vi "TS Manager.vi"(11 "notifier":refnum<notifier>) -> ()   [LabVIEW 2025, in "Config Tool.lvlib"]
doc: "This is the main VI for the configuration editor.Copyright 2017 National Instruments Corporation\n\nLicensed under the Apache License, Version 2.0 (the \"License\"); you may not use this file except in compliance with the License. You may obtain a copy of the License at http://www.apache.org/licenses/LICENSE-2.0\nUnless required by applicable law or agreed to in writing, software distributed under the License is distributed on an \"AS IS\" BASIS, WITHOUT WARRANTIES OR CONDITIONS OF ANY KIND, either express or implied. See the License for the specific language governing permissions and limitations under the License."
uses:
  Controls/StateCluster.ctl
  Users/Public/Documents/Sandia National Labs/TSS Plugin/CEF.lvlibp/Repository/CEF_Repository.lvclass
  Users/Public/Documents/Sandia National Labs/TSS Plugin/CEF.lvlibp/Node/NodeRef.ctl
  Users/Public/Documents/Sandia National Labs/TSS Plugin/CEF.lvlibp/Node/CEF_Node.lvclass
  Users/Public/Documents/Sandia National Labs/TSS Plugin/CEF.lvlibp/Node/StandardEvents.ctl
  Controls/FilePaths.ctl
  Users/Public/Documents/Sandia National Labs/TSS Plugin/CEF.lvlibp/glyph manager/glyph manager.ctl
  <vilib>/Utility/config.llb/Config Data RefNum.ctl
  Controls/AddMessage.ctl
  Controls/MoveMessage.ctl
  Users/Public/Documents/Sandia National Labs/TSS Plugin/CEF.lvlibp/hierarchy repo/CEF_HierarchyRepo.lvclass
  Users/Public/Documents/Sandia National Labs/TSS Plugin/System.lvlibp/System/System.lvclass
  Users/Public/Documents/Sandia National Labs/TSS Plugin/CEF.lvlibp/serializable node/CEF_serializable node.lvclass
  ce7dbd15-68e1-444f-b0a0-607e461cde1a.vi
  TestStandUI/Control Globals.vi
  Users/Public/Documents/Sandia National Labs/TSS Plugin/CEF.lvlibp/Node/ReadChildren.vi
  Users/Public/Documents/Sandia National Labs/TSS Plugin/CEF.lvlibp/Node/ReadNodeClass.vi
  Config Tool.lvlib
  Users/Public/Documents/Sandia National Labs/TSS Plugin/CEF.lvlibp
  <vilib>/Utility/config.llb/NI_LVConfig.lvlib
panel:
  in  "Record":bool
  out "Time":dbl format="%<%H:%M:%S>t"
  in  "Initialize Engines":bool
  in  "File Menu":bool
  in  "TreeView":string(tree)="NID741343233"
  in  "ExecutionView Manager":refnum<k7>(container)
  in  "SequenceFileView Manager":refnum<k7>(container)
  in  "Application Manager":refnum<k7>(container)
  in  "Close Executions Btn":refnum<k7>(container)
  in  "Close Sequence File Btn":refnum<k7>(container)
  in  "Open Sequence File Btn":refnum<k7>(container)
  in  "Run Selected Sequence Btn":refnum<k7>(container)
  in  "Entry Point 2 Btn":refnum<k7>(container)
  in  "Entry Point 1 Btn":refnum<k7>(container)
  in  "Executions ComboBox":refnum<k7>(container) caption="Executions"
  in  "Sequences ComboBox":refnum<k7>(container) caption="Sequences"
  in  "Sequence Files ComboBox":refnum<k7>(container) caption="Sequence Files"
  in  "Execution View":refnum<k7>(container)
  in  "Terminate All Btn":refnum<k7>(container)
  in  "Break/Resume Btn":refnum<k7>(container)
  in  "Terminate/Restart Btn":refnum<k7>(container)
  in  "Report Viewer":refnum<k7>(container)
  in  "TS Pane":bool
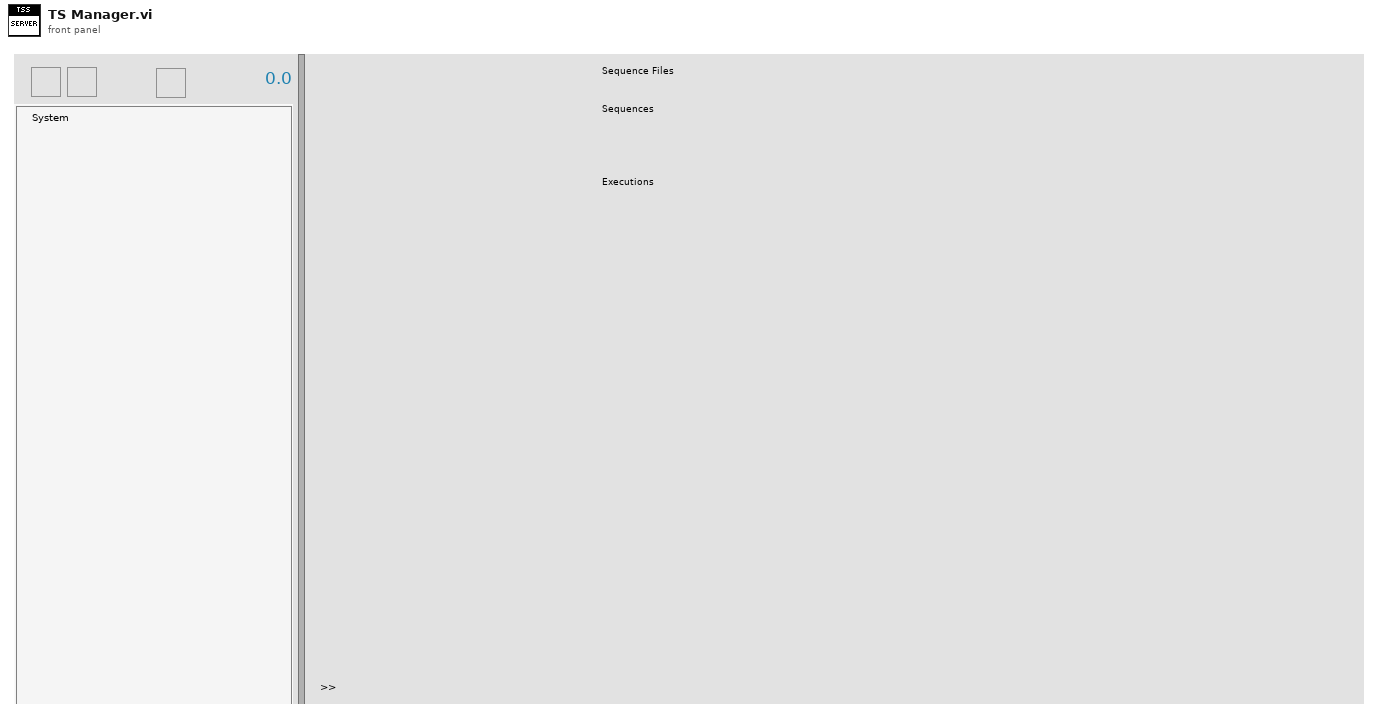
[diagram p1: front panel]
types:
  T1 = typedef "Config Tool.lvlib/StateCluster.ctl" = cluster{"repository":refnum<class "CEF_Repository.lvclass">, "root":T2, "standard events":T3, "paths":T4, "glyph manager":T5, "current path":path, "unsaved changes":bool, "menu":refnum<k9>, "Error Log":refnum<file>, "INI file ref":T6, "Record":bool, "tdms file":refnum<k34>}
  T2 = typedef "CEF.lvlibp/CEF_Node.lvclass/NodeRef.ctl" = refnum<data-value>
  T3 = typedef "CEF.lvlibp/CEF_Node.lvclass/StandardEvents.ctl" = cluster{"user event":refnum<user-event>, "node change":refnum<user-event>, "cache state":refnum<user-event>, "refresh UI":refnum<user-event>, "stop event":refnum<user-event>, "Quit App":refnum<user-event>}
  T4 = typedef "Config Tool.lvlib/FilePaths.ctl" = cluster{"Configuration":path, "Plugin":path, "Glyphs":path, "Data":path, "Error Log":path}
  T5 = typedef "CEF.lvlibp/glyph manager.ctl" = cluster{"search paths":path[], "glyph map":variant, "base glyphs":cluster{"image type":i32, "image depth":i32, "image":u8[], "mask":u8[], "colors":u32[], "Rectangle":cluster{"left":i16, "top":i16, "right":i16, "bottom":i16}}[], "desired overlays":string[]}
  T6 = typedef "NI_LVConfig.lvlib/Config Data RefNum.ctl" = refnum<k1>
  T7 = cluster{"user event":refnum<user-event>, "node change":refnum<user-event>, "cache state":refnum<user-event>, "refresh UI":refnum<user-event>, "stop event":refnum<user-event>, "Quit App":refnum<user-event>}
  T8 = typedef "Config Tool.lvlib/AddMessage.ctl" = cluster{"subNode":string, "Node ID":string}
  T9 = typedef "Config Tool.lvlib/MoveMessage.ctl" = cluster{"node ref":T2, "new parent":T2, "Index":i32}
  T10 = cluster{"Message Name":string, "data string":string}
  T11 = typedef "LVPoint32TypeDef.ctl" = cluster{"Horizontal":i32, "Vertical":i32}
  T12 = cluster{"data name":string, "drag data":variant}[]
  T13 = cluster{"removable":bool, "movable":bool, "duplicate":bool}
  T14 = cluster{"message name":string, "data string":string}
  T15 = enum16{"Start Timer", "Read Time", "Pause", "Resume"}
  T16 = enum16{"open", "open or create", "create or replace", "create", "open (read-only)"}
  T17 = cluster{"search paths":path[], "glyph map":variant, "base glyphs":cluster{"image type":i32, "image depth":i32, "image":u8[], "mask":u8[], "colors":u32[], "Rectangle":cluster{"left":i16, "top":i16, "right":i16, "bottom":i16}}[], "desired overlays":string[]}
  T18 = cluster{"ID":string, "parent ID":string, "node type":string, "text":string, "additional text":string, "glyph":string, "depth":i32, "glyph overlay":string}[]
  T19 = cluster{"ID":string, "parent ID":string, "node type":string, "text":string, "additional text":string, "glyph":string, "depth":i32, "glyph overlay":string}
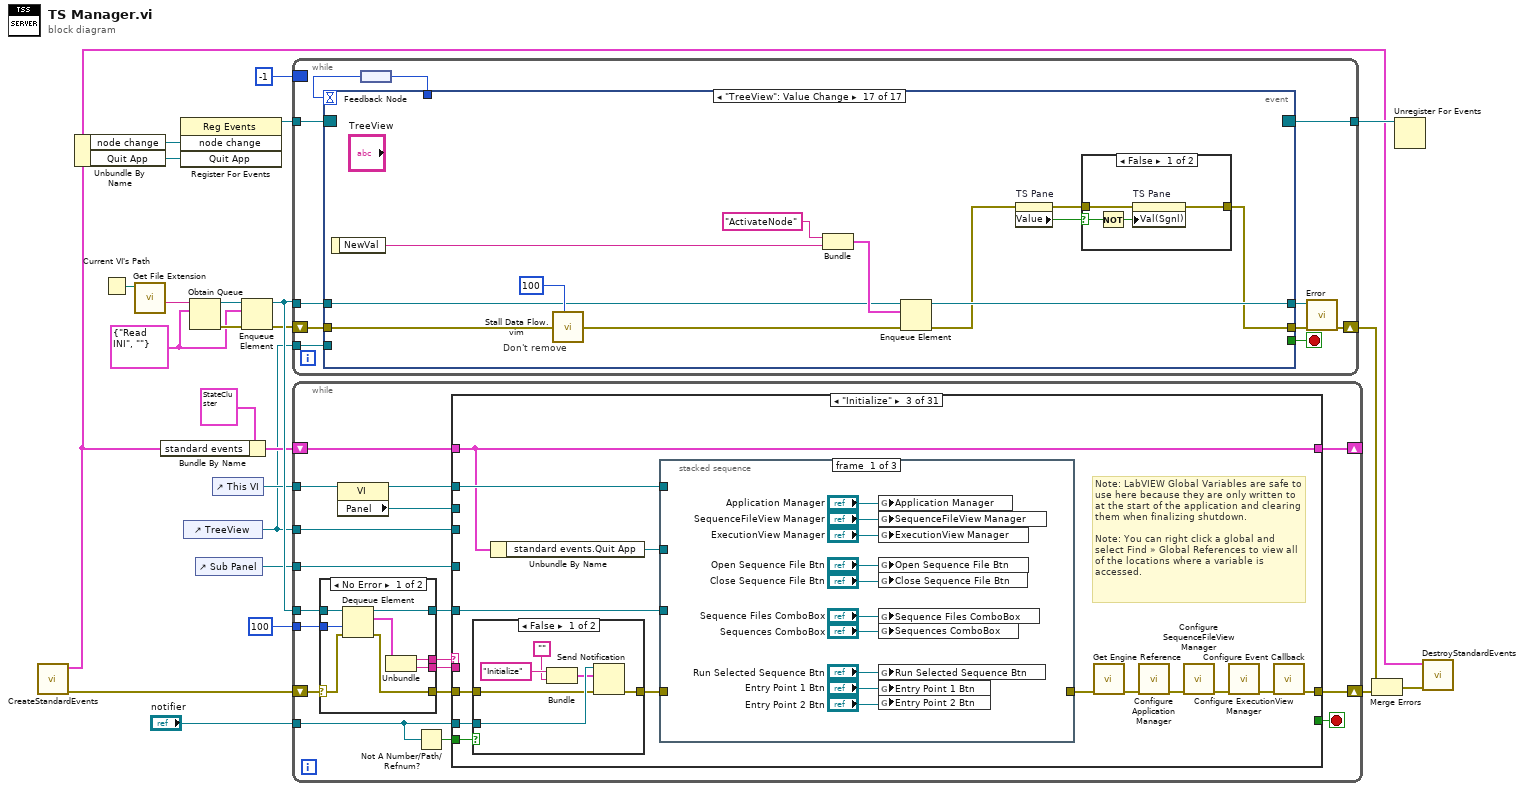
[diagram p0: block diagram]
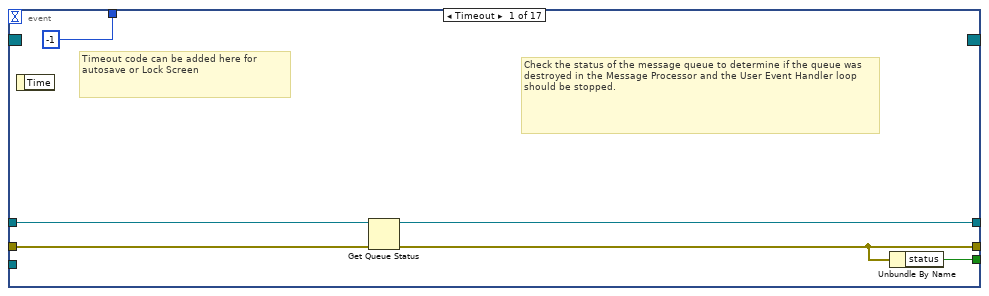
[diagram p2: hidden frame]
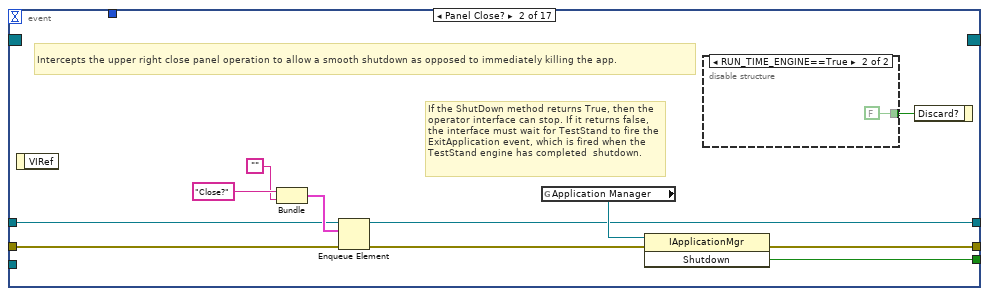
[diagram p3: hidden frame]
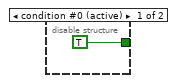
[diagram p4: hidden frame]
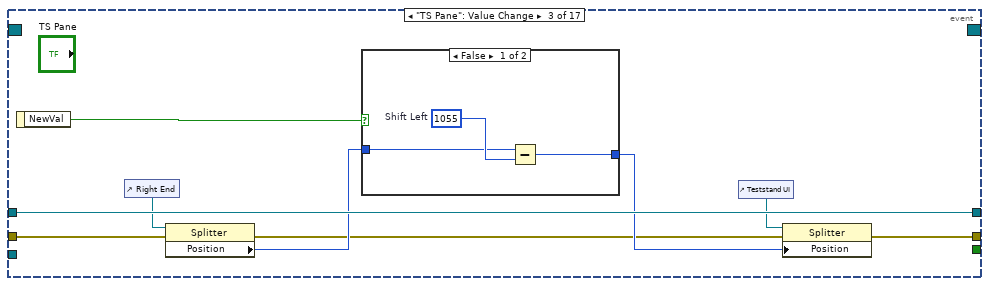
[diagram p5: hidden frame]
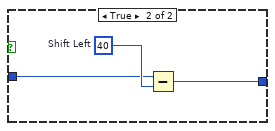
[diagram p6: hidden frame]
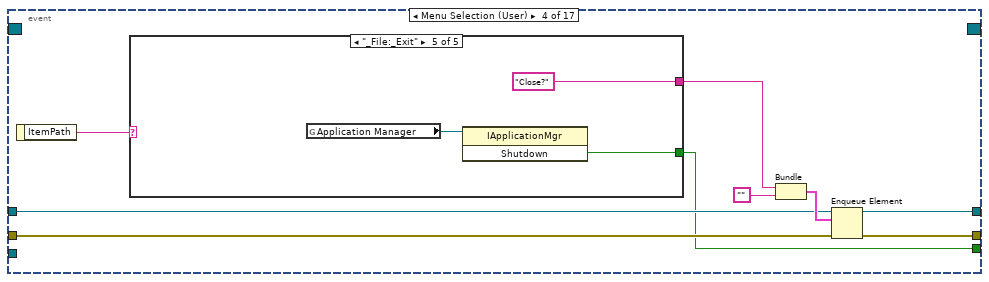
[diagram p7: hidden frame]
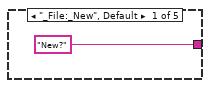
[diagram p8: hidden frame]
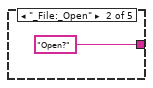
[diagram p9: hidden frame]
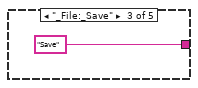
[diagram p10: hidden frame]
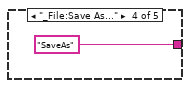
[diagram p11: hidden frame]
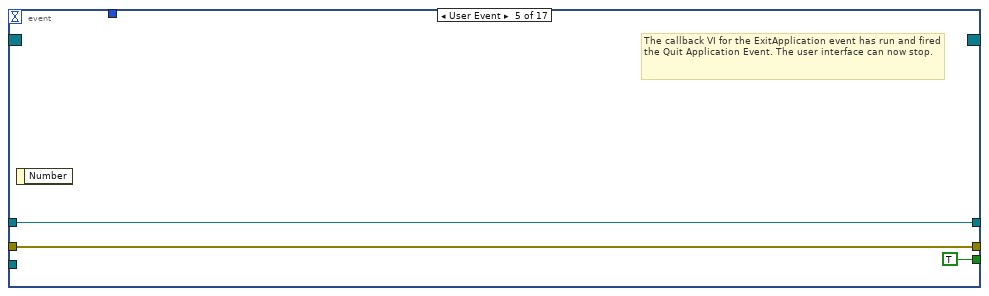
[diagram p12: hidden frame]
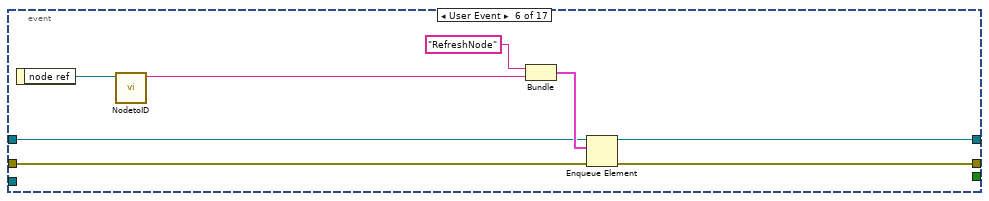
[diagram p13: hidden frame]
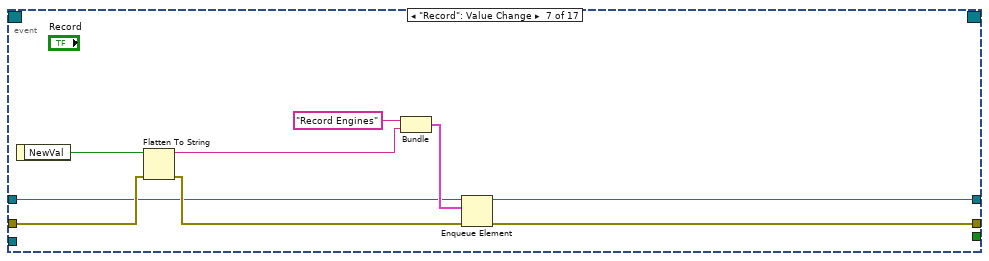
[diagram p14: hidden frame]
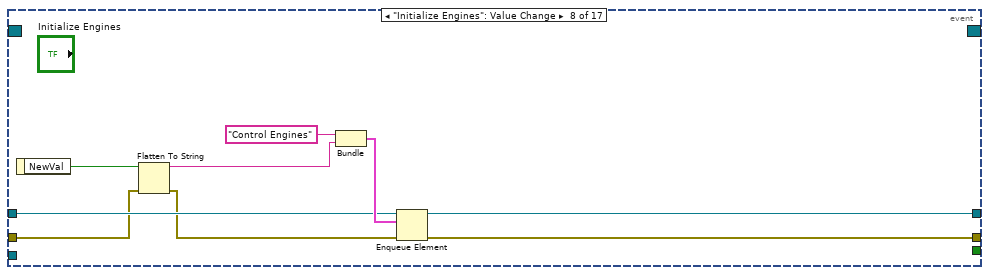
[diagram p15: hidden frame]
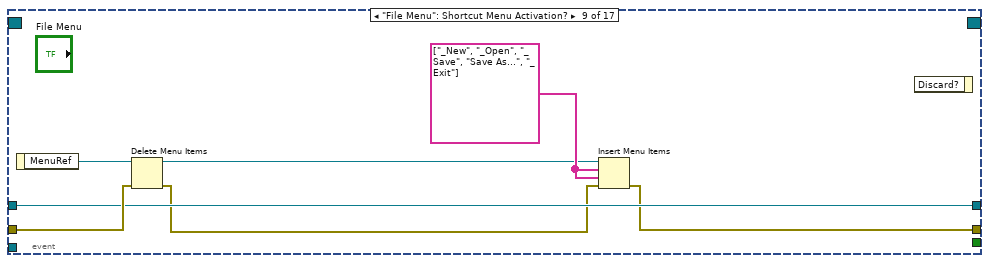
[diagram p16: hidden frame]
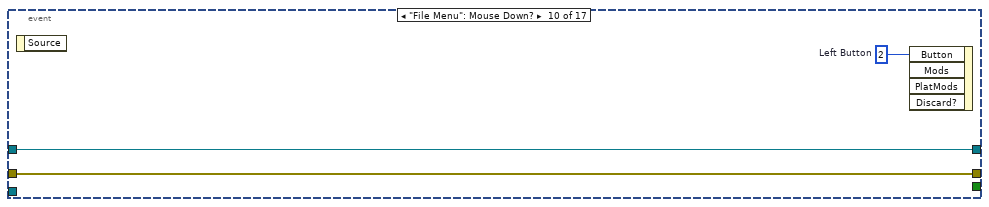
[diagram p17: hidden frame]
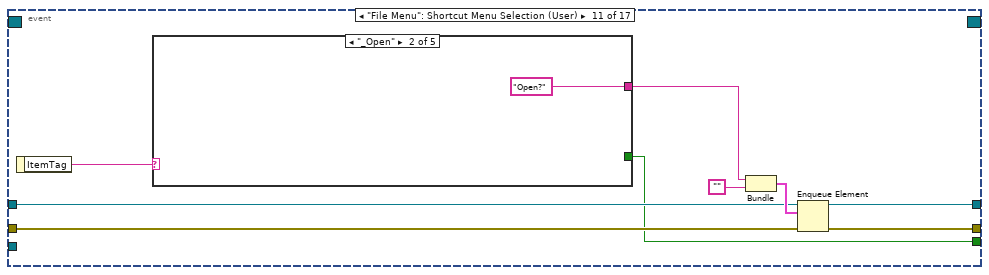
[diagram p18: hidden frame]
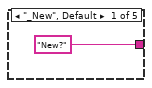
[diagram p19: hidden frame]
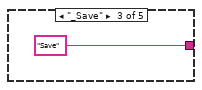
[diagram p20: hidden frame]
diagram:
  w10 = cluster{"message":string, "string":string} {"message"="Read INI", "string"=""}
  n1 = call "CreateStandardEvents.vi"() -> ("error out"=w14:errorcluster, "standard events"=w16:T7)  [unwired: 10 in]
  n2 = Unbundle By Name(w16) -> ("node change"=w15:refnum<user-event>, "Quit App"=w1:refnum<user-event>)
  n3 = Current VI's Path() -> (path=w21:path)
  n4 = call <vilib>:"Get File Extension.vi"("file"=w21) -> ("filename without extension"=w11:string)  [unwired: 6 in, 4 out]
  n5 = Bundle By Name(cluster=T1 {"repository"=refnum, "root"=refnum, "standard events"={"user event"=refnum, "node change"=refnum, "cache state"=refnum, "refresh UI"=refnum, "stop event"=refnum, "Quit App"=refnum}, "paths"={"Configuration"=path "", "Plugin"=path "", "Glyphs"=path "", "Data"=path "", "Error Log"=path ""}, "glyph manager"={"search paths"=[], "glyph map"=variant, "base glyphs"=[], "desired overlays"=[]}, "current path"=path "", "unsaved changes"=FALSE, "menu"=refnum, "Error Log"=refnum, "INI file ref"=refnum, "Record"=FALSE, "tdms file"=refnum} ("state cluster"), "standard events"=w16) -> (w4:T1)
  n6 = register-events(w15, w1) -> (reference out=w2:refnum<event-registration>)  [unwired: 2 in, 1 out]
  n7 = control-ref of="TreeView"() -> (w3:refnum<vi>)
  n8 = Obtain Queue(name (unnamed)=w11, element data type=w10) -> (queue out=w12:refnum<queue>, error out=w13:errorcluster)  [unwired: 3 in, 1 out]
  n9 = control-ref of="Sub Panel"() -> (w5:refnum<vi>)
  n10 = control-ref of="This VI"() -> (w6:refnum<vi>)
  n11 = Enqueue Element(queue=w12, element=w10, error in (no error)=w13) -> (queue out=w9:refnum<queue>, error out=w8:errorcluster)  [unwired: 1 in, 1 out]
  n12 = while "User Interface Event Handler" {
    tunnel: w9 -> [w34]
    tunnel: w3 -> [w29]
    tunnel: w2 -> [w28]
    tunnel: [w27] -> w17
    border: -1 -> [_]
    shift-right: [w31] -> w22
    shift-left: w8 -> [w35]
    stop <- w33 stop-if-true
    n13 = feedback #1() -> (w25:i32)
    n14 = event shown="[16] \"TreeView\": Value Change" {
      selector: w28 -> [_ _ _ _ _ _ _ _ _ _ _ _ _ _ _ _ _]
      dyn-events: [_ _ _ _ _ _ _ _ _ _ _ _ _ _ _ _ _] -> w27
      timeout: w25 -> [_ _ _ _ _ _ _ _ _ _ _ _ _ _ _ _ _]
      tunnel: [w36 w49 _ w71 TRUE ("Shutdown") _ _ _ _ _ w127 _ _ _ _ _ _] -> w33
      tunnel: [w37 w51 w62 w78 w90 w97 w101 w108 w117 w124 w128 w159 w182 w211 w239 w250 w279] -> w32
      tunnel: w35 -> [w38 w45 w57 w72 w90 w91 w103 w110 w123 w124 w129 w150 w181 w210 w237 w251 w290]
      tunnel: w34 -> [w41 w44 w64 w73 w89 w93 w102 w114 w121 w125 w131 w148 w177 w209 w236 w245 w284]
      tunnel: [w40 w43 w64 w77 w89 w92 w100 w113 w121 w125 w130 w148 w176 w209 w236 _ w283] -> w30
      tunnel: w29 -> [_ _ _ _ _ _ _ _ _ _ _ w146 _ _ _ _ _]
      tunnel: [-1 _ _ _ _ _ _ _ _ _ _ _ _ _ _ _ _] -> w26
      event Timeout {
        # "Check the status of the message queue to determine if the queue was destroyed in the Message Processor and the User Event Handler loop should be stopped."
        # "Timeout code can be added here for autosave or Lock Screen"
        n15 = event-data() -> ()  [unwired: 1 in, 1 out]
        n16 = Get Queue Status(queue=w41, error in (no error)=w38) -> (queue out=w40:refnum<queue>, error out=w37:errorcluster)  [unwired: 1 in, 6 out]
        n17 = Unbundle By Name(w37) -> ("status"=w36:bool)
      }
      event Panel Close? {
        # "If the ShutDown method returns True, then the operator interface can stop. If it returns false, the interface must wait for TestStand to fire the ExitApplication event, which is fired when the TestStand engine has completed  shutdown."
        # "Intercepts the upper right close panel operation to allow a smooth shutdown as opposed to immediately killing the app."
        n18 = event-data() -> ()  [unwired: 1 in, 1 out]
        n19 = Bundle("Close?", "") -> (w48:cluster{string, string})  [unwired: 1 in]
        n20 = Enqueue Element(queue=w44, element=w48, error in (no error)=w45) -> (queue out=w43:refnum<queue>, error out=w42:errorcluster)  [unwired: 1 in, 1 out]
        n21 = global read "Control Globals.vi" "Application Manager"() -> (w50:refnum<k7>)
        n22 = global read "Control Globals.vi" "Application Manager"() -> (w52:refnum<k7>)
        n23 = invoke class="IApplicationMgr" method="Shutdown"(reference=w50, error in=w42) -> ()  [unwired: 1 in, 3 out]
        n24 = invoke class="IApplicationMgr" method="Shutdown"(reference=w52) -> (error out=w51:errorcluster, "Shutdown"=w49:bool)  [unwired: 2 in, 1 out]
        n25 = disable-structure shown="RUN_TIME_ENGINE==True" {
          disable-tunnel: [TRUE FALSE] -> w53
          frame condition #0 (active) {
          }
          frame condition #1 {
          }
        }
        n26 = event-data("Discard?"=w53) -> ()  [unwired: 1 in, 1 out]
      }
      event "TS Pane": Value Change {
        n27 = event-data() -> ("NewVal"=w60:bool)  [unwired: 1 in]
        n28 = control-ref of="Right End"() -> (w61:refnum<vi>)
        n29 = property class="Splitter"(reference=w61, error in=w57) -> (error out=w56:errorcluster, "Position"=w59:i32)  [unwired: 1 out]
        n30 = case shown="False" w60 {
          tunnel: w59 -> [w66 w69]
          tunnel: [w65 w68] -> w58
          frame False {
            w67 = 1055  # Shift Left
            n31 = Subtract(x=w66, y=w67) -> (x-y=w65:i32)
          }
          frame True {
            w70 = 40  # Shift Left
            n32 = Subtract(x=w69, y=w70) -> (x-y=w68:i32)
          }
        }
        n33 = control-ref of="Teststand UI"() -> (w63:refnum<vi>)
        n34 = property class="Splitter"(reference=w63, error in=w56, "Position"=w58) -> (error out=w62:errorcluster)  [unwired: 1 out]
      }
      event Menu Selection (User) {
        n35 = event-data() -> ("ItemPath"=w79:string)  [unwired: 1 in]
        n36 = case shown="\"_File:_Exit\"" w79 {
          tunnel: ["New?" ("Message Name") "Open?" ("Message Name") "Save" ("Message Name") "SaveAs" ("Message Name") "Close?" ("Message Name")] -> w75
          tunnel: [_ _ _ _ w84] -> w71
          frame "_File:_New", Default {
          }
          frame "_File:_Open" {
          }
          frame "_File:_Save" {
          }
          frame "_File:Save As..." {
          }
          frame "_File:_Exit" {
            n37 = global read "Control Globals.vi" "Application Manager"() -> (w85:refnum<k7>)
            n38 = global read "Control Globals.vi" "Application Manager"() -> (w86:refnum<k7>)
            n39 = invoke class="IApplicationMgr" method="Shutdown"(reference=w85) -> ("Shutdown"=w84:bool)  [unwired: 2 in, 2 out]
            n40 = invoke class="IApplicationMgr" method="Shutdown"(reference=w86) -> ()  [unwired: 2 in, 3 out]
          }
        }
        n41 = Bundle("Message Name"=w75, "") -> (w74:cluster{"Message Name":string, string})  [unwired: 1 in]
        n42 = Enqueue Element(queue=w73, element=w74, error in (no error)=w72) -> (queue out=w77:refnum<queue>, error out=w78:errorcluster)  [unwired: 1 in, 1 out]
      }
      event User Event {
        # "The callback VI for the ExitApplication event has run and fired the Quit Application Event. The user interface can now stop."
        n43 = event-data() -> ()  [unwired: 1 in, 1 out]
      }
      event User Event {
        n44 = event-data() -> ("node ref"=w98:refnum<data-value>)  [unwired: 1 in]
        n45 = call "NodetoID.vi"("node ref"=w98) -> ("ID"=w94:string)  [unwired: 9 in, 1 out]
        n46 = Bundle("message name"="RefreshNode", "ID"=w94) -> (w95:cluster{"message name":string, "ID":string})  [unwired: 1 in]
        n47 = Enqueue Element(queue=w93, element=w95, error in (no error)=w91) -> (queue out=w92:refnum<queue>, error out=w97:errorcluster)  [unwired: 1 in, 1 out]
      }
      event "Record": Value Change {
        n48 = event-data() -> ("NewVal"=w99:bool)  [unwired: 1 in]
        n49 = Flatten To String(anything=w99, error in (no error)=w103) -> (data string=w105:string, error out=w104:errorcluster)  [unwired: 2 in, 1 out]
        n50 = Bundle("Message Name"="Record Engines", "data string"=w105) -> (w107:T10)  [unwired: 1 in]
        n51 = Enqueue Element(queue=w102, element=w107, error in (no error)=w104) -> (queue out=w100:refnum<queue>, error out=w101:errorcluster)  [unwired: 1 in, 1 out]
      }
      event "Initialize Engines": Value Change {
        n52 = event-data() -> ("NewVal"=w112:bool)  [unwired: 1 in]
        n53 = Flatten To String(anything=w112, error in (no error)=w110) -> (data string=w111:string, error out=w109:errorcluster)  [unwired: 2 in, 1 out]
        n54 = Bundle("Message Name"="Control Engines", "data string"=w111) -> (w116:T10)  [unwired: 1 in]
        n55 = Enqueue Element(queue=w114, element=w116, error in (no error)=w109) -> (queue out=w113:refnum<queue>, error out=w108:errorcluster)  [unwired: 1 in, 1 out]
      }
      event "File Menu": Shortcut Menu Activation? {
        w120 = string[] ["_New", "_Open", "_Save", "Save As...", "_Exit"] ("item names")
        n56 = event-data() -> ("MenuRef"=w122:refnum<k9>)  [unwired: 1 in]
        n57 = Delete Menu Items(6:w123, 9:w122) -> (0:w118:errorcluster, 3:w119:refnum<k9>)  [unwired: 2 in]
        n58 = Insert Menu Items(6:w118, 7:w120, 8:w120, 9:w119) -> (0:w117:errorcluster)  [unwired: 2 in, 2 out]
        n59 = event-data() -> ()  [unwired: 2 in, 1 out]
      }
      event "File Menu": Mouse Down? {
        w126 = u16 2  # Left Button
        n60 = event-data() -> ()  [unwired: 1 in, 1 out]
        n61 = event-data("Button"=w126) -> ()  [unwired: 4 in, 1 out]
      }
      event "File Menu": Shortcut Menu Selection (User) {
        n62 = event-data() -> ("ItemTag"=w135:string)  [unwired: 1 in]
        n63 = case shown="\"_Open\"" w135 {
          tunnel: ["New?" ("Message Name") "Open?" ("Message Name") "Save" ("Message Name") "SaveAs" ("Message Name") "Close?" ("Message Name")] -> w133
          tunnel: [_ _ _ _ w141] -> w127
          frame "_New", Default {
          }
          frame "_Open" {
          }
          frame "_Save" {
          }
          frame "Save As..." {
          }
          frame "_Exit" {
            n64 = global read "Control Globals.vi" "Application Manager"() -> (w142:refnum<k7>)
            n65 = global read "Control Globals.vi" "Application Manager"() -> (w143:refnum<k7>)
            n66 = invoke class="IApplicationMgr" method="Shutdown"(reference=w142) -> ("Shutdown"=w141:bool)  [unwired: 2 in, 2 out]
            n67 = invoke class="IApplicationMgr" method="Shutdown"(reference=w143) -> ()  [unwired: 2 in, 3 out]
          }
        }
        n68 = Bundle("Message Name"=w133, "") -> (w132:cluster{"Message Name":string, string})  [unwired: 1 in]
        n69 = Enqueue Element(queue=w131, element=w132, error in (no error)=w129) -> (queue out=w130:refnum<queue>, error out=w128:errorcluster)  [unwired: 1 in, 1 out]
      }
      event "TreeView": Shortcut Menu Activation? {
        n70 = event-data() -> ("MenuRef"=w149:refnum<k9>, "CtlRef"=w162:refnum<vi>, "Coords"=w161:T11)  [unwired: 1 in]
        n71 = invoke class="Tree (strict)" method="Point To Row Column"(reference=w162, "Point"=w161) -> ("Tag"=w160:string)  [unwired: 6 in, 7 out]
        n72 = property class="Tree (strict)"(reference=w146, error in=w150) -> (error out=w147:errorcluster, "Allow Editing Cells"=w145:bool)  [unwired: 1 out]
        n73 = call "IDtoNode.vi"("error in"=w147, "ID"=w160) -> ("error out"=w155:errorcluster, "invalid Id"=w153:bool, "node ref"=w158:refnum<data-value>)  [unwired: 7 in]
        n74 = Not(x=w153) -> (.not. x?=w144:bool)
        n75 = And(x=w144, y=w145) -> (x .and. y?=w152:bool)
        n76 = case shown="True" w152 {
          tunnel: w158 -> [_ w170]
          tunnel: w149 -> [_ w169]
          tunnel: [_ w168] -> w157
          tunnel: [_ w167] -> w156
          tunnel: w155 -> [w164 w166]
          tunnel: [w164 w166] -> w154
          tunnel: [TRUE ("Discard?") FALSE ("Discard?")] -> w151
          frame False {
          }
          frame True {
            n77 = in-place {
              in-place-border: w169 -> [w173]
              in-place-border: [w171] -> w168
              n78 = in-place-dvr #2(w170) -> (w175:refnum<class "CEF_Node.lvclass">, w172:errorcluster)
              n79 = call-dynamic "ShortcutMenu.vi"("error in"=w172, "menu ref in"=w173, "CEF_Node in"=w175) -> ("error out"=w171:errorcluster, "CEF_Node out"=w174:refnum<class "CEF_Node.lvclass">)  [unwired: 6 in, 1 out]
              n80 = in-place-dvr #2(w174) -> (w167:errorcluster)  [unwired: 1 out]
            }
          }
        }
        n81 = Merge Errors(w156, w157, w154) -> (w159:errorcluster)
        n82 = event-data("Discard?"=w151) -> ()  [unwired: 1 in, 1 out]
      }
      event "TreeView": Shortcut Menu Selection (User) {
        n83 = event-data() -> ("ItemPath"=w184:string, "CtlRef"=w187:refnum<vi>, "Coords"=w188:T11)  [unwired: 1 in]
        n84 = invoke class="Tree (strict)" method="Point To Row Column"(reference=w187, "Point"=w188) -> ("Tag"=w183:string)  [unwired: 6 in, 7 out]
        n85 = Match Pattern(string=w184, regular expression=":") -> (before substring=w186:string, after substring=w185:string)  [unwired: 1 in, 2 out]
        n86 = case shown="\"Export\"" w186 {
          selector: w186 -> [w192 _ _ _ _ _]
          tunnel: w185 -> [_ _ _ w202 _ _]
          tunnel: w183 -> [w193 w195 w197 w203 w205 w208]
          tunnel: ["CustomMenuAction" ("Message Name") "RemoveNode" ("Message Name") "Duplicate" ("Message Name") "AddNode" ("Message Name") "Import Engine" ("Message Name") "Export Engine" ("Message Name")] -> w179
          tunnel: [w190 w195 w197 w199 w205 w208] -> w180
          frame Default {
            # "Right click menu"
            n87 = Concatenate Strings(w192, ":" ("string"), w193) -> (w190:string)
          }
          frame "Remove" {
          }
          frame "Duplicate" {
          }
          frame "Add" {
            n88 = Bundle By Name(cluster=T8 {"subNode"="", "Node ID"=""} ("input cluster"), "subNode"=w202, "Node ID"=w203) -> (w200:T8)
            n89 = Flatten To String(anything=w200) -> (data string=w199:string)  [unwired: 3 in, 2 out]
          }
          frame "Import" {
          }
          frame "Export" {
          }
        }
        n90 = Bundle("Message Name"=w179, "Tag"=w180) -> (w178:cluster{"Message Name":string, "Tag":string})  [unwired: 1 in]
        n91 = Enqueue Element(queue=w177, element=w178, error in (no error)=w181) -> (queue out=w176:refnum<queue>, error out=w182:errorcluster)  [unwired: 1 in, 1 out]
      }
      event "TreeView": Drag Starting? {
        n92 = event-data() -> ("Data"=w218:T12, "CtlRef"=w220:refnum<vi>, "Coords"=w219:T11)  [unwired: 1 in]
        n93 = invoke class="Tree (strict)" method="Point To Row Column"(reference=w220, "Point"=w219) -> ("Tag"=w217:string)  [unwired: 6 in, 7 out]
        n94 = call "IDtoNode.vi"("error in"=w210, "ID"=w217) -> ("error out"=w212:errorcluster, "invalid Id"=w216:bool, "node ref"=w215:refnum<data-value>)  [unwired: 7 in]
        n95 = case shown="False" w216 {
          tunnel: w215 -> [w228 _]
          tunnel: [w225 TRUE ("Removable")] -> w213
          tunnel: w212 -> [w224 w234]
          tunnel: [w221 w234] -> w211
          frame False {
            n96 = in-place {
              in-place-border: [w231] -> w227
              in-place-border: w224 -> [w230]
              in-place-border: [w229] -> w223
              n97 = in-place-dvr #3(w228) -> (w233:refnum<class "CEF_Node.lvclass">)  [unwired: 1 out]
              n98 = call-dynamic "EditOptions.vi"("error in"=w230, "CEF_Node in"=w233) -> ("error out"=w229:errorcluster, "edit options"=w231:T13, "CEF_Node out"=w232:refnum<class "CEF_Node.lvclass">)  [unwired: 6 in, 1 out]
              n99 = in-place-dvr #3(w232) -> (w222:errorcluster)  [unwired: 1 out]
            }
            n100 = Unbundle By Name(w227) -> ("movable"=w226:bool)
            n101 = Merge Errors(w222, w223) -> (w221:errorcluster)
            n102 = Not(x=w226) -> (.not. x?=w225:bool)
          }
          frame True {
          }
        }
        n103 = event-data("Data"=w218, "Drag Mode"=enum32{"copy or move", "copy only", "move only"}."move only", "Discard?"=w213) -> ()  [unwired: 1 in, 1 out]
      }
      event "TreeView": event type 3.0.xa000003a {
        n104 = event-data() -> ("CtlRef"=w244:refnum<vi>, "Coords"=w241:T11)  [unwired: 1 in]
        n105 = invoke class="Tree (strict)" method="Point To Row Column"(reference=w244, "Point"=w241) -> (reference out=w243:refnum<vi>, "Tag"=w242:string)  [unwired: 6 in, 6 out]
        n106 = call "ValidDragDrop.vi"("error in"=w237, "Reorder"=TRUE, "drag over"=w242, "Tree Ref in"=w243) -> ("Error Out"=w239:errorcluster, "Accepted"=w240:bool)  [unwired: 6 out]
        n107 = event-data("Accepted?"=w240) -> ()  [unwired: 1 in, 1 out]
      }
      event "TreeView": Drop {
        n108 = event-data() -> ("CtlRef"=w262:refnum<vi>, "Coords"=w261:T11)  [unwired: 1 in]
        n109 = invoke class="Tree (strict)" method="Point To Row Column"(reference=w262, "Point"=w261) -> (reference out=w260:refnum<vi>, "Tag"=w257:string)  [unwired: 6 in, 6 out]
        n110 = call "ValidDragDrop.vi"("error in"=w251, "Reorder"=TRUE, "drag over"=w257, "Tree Ref in"=w260) -> ("Error Out"=w249:errorcluster, "Accepted"=w255:bool, "Drag"=w259:string, "Tree Ref out"=w264:refnum<vi>, "Moved Node"=w253:refnum<data-value>, "Position"=w252:i32, "Parent Node"=w254:refnum<data-value>, "Parent"=w256:string)
        n111 = case shown="True" w255 {
          tunnel: w259 -> [_ w276]
          tunnel: w264 -> [_ w278]
          tunnel: [_ TRUE] -> w263
          tunnel: w256 -> [_ w275]
          tunnel: w253 -> [_ w274]
          tunnel: w254 -> [_ w273]
          tunnel: w252 -> [_ w272]
          tunnel: ["Idle" ("message name") "Move" ("message name")] -> w248
          tunnel: [_ w267] -> w247
          frame False {
          }
          frame True {
            n112 = invoke class="Tree (strict)" method="Edit Tree Items.Move Item"(reference=w278, "tag"=w276, "New Parent"=w275, "New Position"=0, "Carry Children"=FALSE ("Carry Children?")) -> ()  [unwired: 2 in, 7 out]
            n113 = Bundle By Name(cluster=T9 {"node ref"=refnum, "new parent"=refnum, "Index"=0}, "Index"=w272, "node ref"=w274, "new parent"=w273) -> (w269:T9)
            n114 = Flatten To String(anything=w269) -> (data string=w267:string)  [unwired: 3 in, 2 out]
          }
        }
        n115 = Bundle("message name"=w248, "data string"=w247) -> (w246:T14)  [unwired: 1 in]
        n116 = Enqueue Element(queue=w245, element=w246, error in (no error)=w249) -> (error out=w250:errorcluster)  [unwired: 1 in, 2 out]
        n117 = event-data("Accepted?"=w263) -> ()  [unwired: 1 in, 1 out]
      }
      event "TreeView": Value Change {
        # "Don't remove"
        n118 = event-data() -> ("NewVal"=w286:string)  [unwired: 1 in]
        n119 = call "Stall Data Flow.vim"("value in"=w290, "milliseconds to wait"=u32 100) -> ("value out"=w289:errorcluster)  [unwired: 1 out]
        n120 = Bundle("Message Name"="ActivateNode", "NewVal"=w286) -> (w285:cluster{"Message Name":string, "NewVal":string})  [unwired: 1 in]
        n121 = Enqueue Element(queue=w284, element=w285, error in (no error)=w289) -> (queue out=w283:refnum<queue>, error out=w282:errorcluster)  [unwired: 1 in, 1 out]
        n122 = property on="TS Pane" class="Bool (strict)"(error in=w282) -> (error out=w280:errorcluster, "Value"=w281:bool)  [unwired: 1 in, 1 out]
        n123 = case shown="False" w281 {
          selector: w281 -> [w292 _]
          tunnel: w280 -> [w294 w295]
          tunnel: [w293 w295] -> w279
          frame False {
            n124 = Not(x=w292) -> (.not. x?=w291:bool)
            n125 = property on="TS Pane" class="Bool (strict)"(error in=w294, "Val(Sgnl)"=w291) -> (error out=w293:errorcluster)  [unwired: 1 in, 1 out]
          }
          frame True {
          }
        }
      }
    }
    n126 = feedback-in #1(w26) -> ()
    n127 = call "Error.vi"("error in (no error)"=w32, "main queue"=w30) -> ("error out"=w31:errorcluster)  [unwired: 9 in]
  }
  n128 = while "Message Processor" {
    shift-right: [w312] -> _
    shift-left: w4 -> [w313]
    tunnel: w9 -> [w308]
    shift-right: [w299] -> w24
    shift-left: w14 -> [w304]
    tunnel: "notifier" -> [w310]
    tunnel: 100 ("timeout (1 ms)") -> [w306]
    tunnel: w6 -> [w298]
    tunnel: w3 -> [w301]
    tunnel: w5 -> [w300]
    stop <- w305 stop-if-true
    n129 = case shown="No Error" w304 {
      selector: w304 -> [w317 w324]
      tunnel: [w321 _] -> w309
      tunnel: w308 -> [w320 w325]
      tunnel: [w319 w325] -> w307
      tunnel: w306 -> [w318 _]
      tunnel: [w315 "Error" ("message")] -> w303
      tunnel: [w314 w323] -> w302
      frame No Error {
        n130 = Dequeue Element(queue=w320, timeout in ms (-1)=w318, error in (no error)=w317) -> (queue out=w319:refnum<queue>, element=w316:cluster{"message":string, "string":string}, error out=w321:errorcluster)  [unwired: 1 out]
        n131 = Unbundle(w316) -> ("message"=w315:string, "string"=w314:string)
      }
      frame Error {
        n132 = Flatten To String(anything=w324) -> (data string=w323:string)  [unwired: 3 in, 2 out]
      }
    }
    n133 = property class="VI"(reference=w298) -> (reference out=w297:refnum<vi>, "Panel"=w296:refnum<vi>)  [unwired: 1 in, 1 out]
    n134 = Not A Number/Path/Refnum?(number/path/refnum=w310) -> (NaN/Path/Refnum?=w311:bool)
    n135 = case shown="\"Initialize\"" w303 {
      selector: w303 -> [_ _ _ _ _ _ w581 _ _ _ _ w646 _ _ _ _ _ _ _ _ _ _ _ _ _ _ _ _ _ _ _]
      tunnel: w302 -> [_ _ _ _ _ w513 _ _ _ _ _ _ w670 _ _ _ _ w852 w864 w899 w961 w977 w1011 w1030 w1075 w1091 _ w1115 w1146 w1215 w1253]
      tunnel: w309 -> [w327 w334 w364 w427 w451 w514 w585 w592 w606 w623 w636 w648 w678 w706 w774 w812 w831 w853 w863 w893 w970 w981 w1008 w1028 w1072 w1090 w1105 w1116 w1151 w1216 w1254]
      tunnel: [w327 w338 w360 w425 w444 w516 w578 w586 w607 w614 w636 w650 w668 w711 w777 w814 w831 w838 w873 w900 w956 w974 w995 w1033 w1067 w1093 w1105 w1110 w1154 w1204 w1250] -> w299
      tunnel: [w326 w349 w359 w436 w447 w515 w579 w602 w612 w632 w635 w639 w684 w726 w781 w813 w830 w861 w868 w898 w971 w975 w1013 w1037 w1070 w1095 w1104 w1108 w1155 w1222 w1248] -> w312
      tunnel: w313 -> [w326 w347 w359 w420 w448 w515 w579 w602 w612 w632 w635 w639 w683 w727 w782 w816 w830 w860 w869 w898 w968 w973 w1014 w1037 w1069 w1092 w1104 w1109 w1156 w1222 w1249]
      tunnel: w307 -> [_ w337 w367 w432 w446 w506 _ w595 w604 w622 _ w643 w679 w709 _ _ _ w834 _ w897 _ _ _ w1034 w1059 w1085 _ _ w1158 w1207 w1247]
      tunnel: w310 -> [_ w344 w365 w422 w453 w504 _ _ _ _ _ _ w680 _ _ _ _ _ _ w891 _ _ w999 _ _ w1077 _ _ _ w1217 _]
      tunnel: w311 -> [_ w342 w366 w421 w452 w503 _ _ _ _ _ _ w671 w707 _ _ _ _ _ _ _ _ w1000 _ _ _ _ _ _ w1205 _]
      tunnel: [_ _ _ _ _ _ _ _ _ TRUE ("Exit") _ _ _ _ _ _ _ _ _ _ _ _ _ _ _ _ _ _ _ _ _] -> w305
      tunnel: w297 -> [_ _ w371 w429 w449 _ w576 _ _ w613 _ _ _ _ _ _ _ _ _ _ _ _ w1001 _ _ _ _ _ _ _ _]
      tunnel: w301 -> [_ w331 _ w416 w450 _ _ _ _ _ _ _ _ _ _ _ _ w832 w862 w894 w954 w972 w1004 _ _ w1081 _ _ _ w1218 w1246]
      tunnel: w300 -> [_ _ _ _ _ _ _ _ _ w628 _ _ _ _ _ _ _ _ _ _ _ _ w1003 w1027 _ _ _ _ _ _ _]
      tunnel: w296 -> [_ _ _ _ _ _ _ w600 _ w627 _ _ _ _ _ _ _ _ _ _ _ _ _ w1026 _ _ _ _ _ _ _]
      frame "------------Generic Operations------------" {
        # "Dummy case to add a seperation in the Case Structure menu"
      }
      frame "Read INI" {
        w335 = "Test Config.ini"
        n136 = Bundle("Initialize", "") -> (w340:cluster{string, string})  [unwired: 1 in]
        n137 = Enqueue Element(queue=w337, element=w340, error in (no error)=w334) -> (error out=w333:errorcluster)  [unwired: 1 in, 2 out]
        n138 = case shown="False" w342 {
          tunnel: w344 -> [w356 _]
          tunnel: w333 -> [w353 w357]
          tunnel: [w352 w357] -> w330
          tunnel: w335 -> [w351 _]
          frame False {
            n139 = Bundle("notification"="Read INI", w351) -> (w354:cluster{"notification":string, string})  [unwired: 1 in]
            n140 = Send Notification(notification=w354, notifier=w356, error in (no error)=w353) -> (error out=w352:errorcluster)  [unwired: 1 out]
          }
          frame True {
          }
        }
        n141 = invoke class="Tree (strict)" method="Edit Tree Items.Delete"(reference=w331, "Delete Children"=TRUE ("Delete Children?")) -> (reference out=w329:refnum<vi>)  [unwired: 3 in, 4 out]
        n142 = call <vilib>:"Application Directory.vi"() -> ("Application Directory"=w346:path)
        n143 = Build Path(base path=w346, name or relative path=w335) -> (appended path=w350:path)
        n144 = invoke class="Tree (strict)" method="Custom Item Symbols.Revert Symbols"(reference=w329, error in=w330) -> (error out=w328:errorcluster)  [unwired: 1 in, 2 out]
        n145 = call "Read INI File.vi"("INI File"=w350) -> ("File paths"=w345:T4, "INI refnum"=w348:T6)  [unwired: 8 in, 1 out]
        n146 = Unbundle By Name(w345) -> ("Error Log"=w343:path)
        n147 = call "Log Error.vi"("Error In"=w328, "Log Path"=w343) -> ("Error Out"=w338:errorcluster, "Log refnum out"=w336:refnum<file>)  [unwired: 8 in]
        n148 = Bundle By Name(cluster=w347, "INI file ref"=w348, "paths"=w345, "Error Log"=w336) -> (w349:T1)
      }
      frame "Initialize" {
        # "Note: LabVIEW Global Variables are safe to use here because they are only written to at the start of the application and clearing them when finalizing shutdown. \n \nNote: You can right click a global and select Find » Global References to view all of the locations where a variable is accessed."
        n149 = case shown="False" w366 {
          tunnel: w365 -> [w377 _]
          tunnel: w364 -> [w374 w378]
          tunnel: [w373 w378] -> w363
          frame False {
            n150 = Bundle("notification"="Initialize", "") -> (w375:cluster{"notification":string, string})  [unwired: 1 in]
            n151 = Send Notification(notification=w375, notifier=w377, error in (no error)=w374) -> (error out=w373:errorcluster)  [unwired: 1 out]
          }
          frame True {
          }
        }
        n152 = Unbundle By Name(w359) -> ("standard events.Quit App"=w358:refnum<user-event>)
        n153 = stacked-sequence {
          tunnel: w371 -> [_ _ w407]
          tunnel: w358 -> [_ _ w406]
          tunnel: w367 -> [_ _ w402]
          tunnel: w363 -> [_ _ w401]
          tunnel: [_ _ w397] -> w362
          frame #0 {
            n154 = global write "Control Globals.vi" "Application Manager"("Application Manager") -> ()
            n155 = global write "Control Globals.vi" "SequenceFileView Manager"("SequenceFileView Manager") -> ()
            n156 = global write "Control Globals.vi" "ExecutionView Manager"("ExecutionView Manager") -> ()
            n157 = global write "Control Globals.vi" "Open Sequence File Btn"("Open Sequence File Btn") -> ()
            n158 = global write "Control Globals.vi" "Close Sequence File Btn"("Close Sequence File Btn") -> ()
            n159 = global write "Control Globals.vi" "Sequence Files ComboBox"("Sequence Files ComboBox") -> ()
            n160 = global write "Control Globals.vi" "Sequences ComboBox"("Sequences ComboBox") -> ()
            n161 = global write "Control Globals.vi" "Run Selected Sequence Btn"("Run Selected Sequence Btn") -> ()
            n162 = global write "Control Globals.vi" "Entry Point 1 Btn"("Entry Point 1 Btn") -> ()
            n163 = global write "Control Globals.vi" "Entry Point 2 Btn"("Entry Point 2 Btn") -> ()
          }
          frame #1 {
            n164 = global write "Control Globals.vi" "Executions ComboBox"("Executions ComboBox") -> ()
            n165 = global write "Control Globals.vi" "Execution View"("Execution View") -> ()
            n166 = global write "Control Globals.vi" "Report Viewer"("Report Viewer") -> ()
            n167 = global write "Control Globals.vi" "Break/Resume Btn"("Break/Resume Btn") -> ()
            n168 = global write "Control Globals.vi" "Terminate/Restart Btn"("Terminate/Restart Btn") -> ()
            n169 = global write "Control Globals.vi" "Close Executions Btn"("Close Executions Btn") -> ()
            n170 = global write "Control Globals.vi" "Terminate All Btn"("Terminate All Btn") -> ()
          }
          frame #2 {
            n171 = global write "Control Globals.vi" "Top level VI"(w407) -> ()
            n172 = global write "Control Globals.vi" "Quit Application Event"(w406) -> ()
            n173 = Bundle("Start Application", "") -> (w405:cluster{string, string})  [unwired: 1 in]
            n174 = Enqueue Element(queue=w402, element=w405, error in (no error)=w401) -> (error out=w400:errorcluster)  [unwired: 1 in, 2 out]
            n175 = property on="TS Pane" class="Bool (strict)"(error in=w400, "Val(Sgnl)"=FALSE ("Value (Signaling)")) -> (error out=w398:errorcluster)  [unwired: 1 in, 1 out]
            n176 = property on="Record" class="Bool (strict)"(error in=w398, "Value"=FALSE ("Record")) -> (error out=w397:errorcluster)  [unwired: 1 in, 1 out]
          }
        }
        n177 = call "Get Engine Reference.vi"("error in (no error)"=w362) -> ("error out"=w368:errorcluster)  [unwired: 10 in]
        n178 = call "Configure Application Manager.vi"("error in (no error)"=w368) -> ("error out"=w370:errorcluster)  [unwired: 10 in]
        n179 = call "Configure SequenceFileView Manager.vi"("error in (no error)"=w370) -> ("error out"=w369:errorcluster)  [unwired: 10 in]
        n180 = call "Configure ExecutionView Manager.vi"("error in"=w369) -> ("error out"=w361:errorcluster)  [unwired: 10 in]
        n181 = call "Configure Event Callback.vi"("error in (no error)"=w361) -> ("error out"=w360:errorcluster)  [unwired: 10 in]
      }
      frame "Start Application" {
        w428 = TRUE ("Front Panel Window:Is Frontmost")
        n182 = Unbundle By Name(w420) -> ("paths.Glyphs"=w419:path)
        n183 = Bundle("New", "") -> (w435:cluster{string, string})  [unwired: 1 in]
        n184 = property class="VI"(reference=w429, "Front Panel.TitleBarVis"=w428, "Front Panel.IsFrontmost"=w428) -> (reference out=w431:refnum<vi>, error out=w430:errorcluster)  [unwired: 1 in]
        n185 = Enqueue Element(queue=w432, element=w435, error in (no error)=w427) -> (error out=w423:errorcluster)  [unwired: 1 in, 2 out]
        n186 = case shown="False" w421 {
          tunnel: w422 -> [w442 _]
          tunnel: w423 -> [w439 w443]
          tunnel: [w438 w443] -> w417
          frame False {
            n187 = Bundle("notification"="Start", "") -> (w440:cluster{"notification":string, string})  [unwired: 1 in]
            n188 = Send Notification(notification=w440, notifier=w442, error in (no error)=w439) -> (error out=w438:errorcluster)  [unwired: 1 out]
          }
          frame True {
          }
        }
        n189 = invoke class="VI" method="Default Vals.Reinit All"(reference=w431, error in=w430) -> (reference out=w412:refnum<vi>)  [unwired: 1 in, 2 out]
        n190 = call "create glyph manager.vi"("error in"=w417, "tree ref (for default symbols)"=w416) -> ("error out"=w411:errorcluster, "glyph manager"=w410:T17)  [unwired: 8 in]
        n191 = call "update tree control.vi"("error in"=w411, "tree reference"=w416, "glyph manager in"=w410) -> ("error out"=w408:errorcluster, "glyph manager out"=w409:T17)  [unwired: 7 in]
        n192 = call "add search path.vi"("error in"=w408, "search path"=w419, "glyph manager in"=w409) -> ("error out"=w415:errorcluster, "glyph manager out"=w418:T17)  [unwired: 7 in]
        n193 = Current VI's Menubar() -> (w414:refnum<k9>)
        n194 = global read "Control Globals.vi" "Application Manager"() -> (w424:refnum<k7>)
        n195 = call "MenuOptions.vi"("VI ref"=w412, "menu ref in"=w414) -> ("menu ref out"=w413:refnum<k9>)  [unwired: 8 in, 1 out]
        n196 = call <vilib>:"TestStand - Set TestStand Application Window.vi"("error in (no error)"=w415, "VI Refnum (Caller's Refnum)"=w412, "Application Manager"=w424) -> ("error out"=w426:errorcluster)  [unwired: 8 out]
        n197 = invoke class="IApplicationMgr" method="Start"(reference=w424, error in=w426) -> (error out=w425:errorcluster)  [unwired: 1 in, 2 out]
        n198 = Bundle By Name(cluster=w420, "glyph manager"=w418, "menu"=w413) -> (w436:T1)
      }
      frame "", "Idle" {
        n199 = case shown="True" w452 {
          tunnel: w453 -> [_ _]
          tunnel: w451 -> [w455 w468]
          tunnel: [w455 w464] -> w445
          tunnel: w450 -> [_ w457]
          tunnel: w449 -> [_ w466]
          tunnel: w448 -> [w454 w469]
          tunnel: [w454 w469] -> w447
          tunnel: w446 -> [_ w463]
          frame False {
          }
          frame True {
            n200 = Unbundle By Name(w469) -> ("current path"=w470:path, "root"=w460:T2, "Record"=w459:bool, "tdms file"=w456:refnum<k34>)
            n201 = property class="Tree (strict)"(reference=w457, error in=w468) -> (reference out=w475:refnum<vi>, error out=w467:errorcluster, "All Tags"=w477:string[], "NumRows"=w474:u32)
            n202 = property class="NISE_CEF_Node"(reference=w460) -> ("DataAccess:Children"=w462:refnum<data-value>[])  [unwired: 1 in, 2 out]
            n203 = Array Size(array=w477) -> (size(s)=w473:i32)
            n204 = To Unsigned Long Integer(number=w473) -> (unsigned 32bit integer=w476:u32)
            n205 = Path To String(path=w470) -> (string=w471:string)
            n206 = Greater Or Equal?(x=w476, y=w474) -> (x >= y?=w472:bool)
            n207 = property class="VI"(reference=w466, "Front Panel.Title"=w471) -> ()  [unwired: 1 in, 2 out]
            n208 = Index Array(array=w462) -> (element=w461:refnum<data-value>)  [unwired: 1 in]
            n209 = property class="Tree (strict)"(reference=w475, error in=w467, "VScrollVis"=w472) -> (error out=w465:errorcluster)  [unwired: 1 out]
            n210 = property class="NISE_CEF_Node"(reference=w461) -> ("DataAccess:Children"=w458:refnum<data-value>[])  [unwired: 1 in, 2 out]
            n211 = case shown="True" w459 {
              tunnel: w465 -> [w478 w486]
              tunnel: [w478 w485] -> w464
              tunnel: w463 -> [_ w484]
              tunnel: w458 -> [_ w483]
              tunnel: w457 -> [_ w482]
              tunnel: w456 -> [_ w481]
              frame False {
              }
              frame True {
                n212 = for {
                  tunnel: w483 -> [w492] mode=indexing
                  shift-right: [w490] -> w485
                  shift-left: w486 -> [w491]
                  tunnel: w482 -> [w489]
                  tunnel: w484 -> [w488]
                  tunnel: w481 -> [w487]
                  n213 = in-place {
                    in-place-border: w491 -> [w496]
                    in-place-border: [w497] -> w490
                    in-place-border: w489 -> [w499]
                    in-place-border: w488 -> [w494]
                    in-place-border: w487 -> [w493]
                    n214 = in-place-dvr #4(w492) -> (w500:refnum<class "CEF_Node.lvclass">)  [unwired: 1 out]
                    n215 = call-dynamic "MenuHandler.vi"("tree control"=w499, "main queue"=w494, "error in"=w496, "parameters"=w493, "menu string"="Record", "CEF_Node in"=w500) -> ("error out"=w497:errorcluster, "CEF_Node out"=w498:refnum<class "CEF_Node.lvclass">)  [unwired: 2 in, 2 out]
                    n216 = in-place-dvr #4(w498) -> ()  [unwired: 2 out]
                  }
                }
                n217 = call "Timing FGV.vi"("Timer Mode"=T15."Read Time") -> ("Elapsed Time (s.ms)"=→"Time":dbl)  [unwired: 8 in, 2 out]
              }
            }
          }
        }
        n218 = call <vilib>:"Unset Busy.vi"("error in (no error)"=w445) -> ("error out"=w444:errorcluster)  [unwired: 10 in]
      }
      frame "Error" {
        n219 = Unflatten From String(type=errorcluster {"status"=FALSE, "code"=0, "source"=""} ("error out"), binary string=w513, error in (no error)=w514) -> (value=w511:errorcluster)  [unwired: 2 in, 2 out]
        n220 = Get Date/Time In Seconds() -> (seconds since 1Jan1904=w519:timestamp)
        n221 = Unbundle By Name(w511) -> ("code"=w502:i32)
        n222 = Format Date/Time String(time format string (%c)="%H:%M:%S", seconds (now)=w519) -> (date/time string=w510:string)  [unwired: 1 in]
        n223 = Unbundle By Name(w515) -> ("Error Log"=w509:refnum<file>)
        n224 = case shown="42..44" w502 {
          tunnel: w511 -> [w526 w528 w531 w538 w541 w543 w548 w556 w557 w562 w567]
          tunnel: [w527 w529 w533 w537 w540 w544 w546 w553 w558 w560 w565] -> w501
          tunnel: w506 -> [_ _ _ _ _ _ _ _ _ _ w575]
          tunnel: [w526 _ w530 w536 w539 w542 w545 _ w557 w559 w566] -> w505
          tunnel: w504 -> [_ _ _ _ _ _ _ _ _ _ w568]
          tunnel: w503 -> [_ _ _ _ _ _ _ _ _ _ _]
          frame 538504, 538505 {
            n225 = Unbundle By Name(w526) -> ("source"=w527:string)
          }
          frame Default {
            n226 = call <vilib>:"Simple Error Handler.vi"("error in (no error)"=w528) -> ()  [unwired: 4 in, 5 out]
            n227 = Unbundle By Name(w528) -> ("source"=w529:string)
          }
          frame -2147220623, -2147220621, -2147220364, 56, 63, 537053 {
            n228 = Unbundle By Name(w531) -> ("source"=w535:string)
            n229 = Concatenate Strings(w535, "\n", "*Note : Problem communicating with remote device.  Make sure a valid device is selected and that the IP address is correct.\n" ("message")) -> (w533:string)
            n230 = Bundle By Name(cluster=w531, "source"=w533) -> (w530:errorcluster)
          }
          frame 1000 {
            w537 = "Invoke error : Abort VI at Subpanel." ("message")
            n231 = Bundle By Name(cluster=w538, "source"=w537) -> (w536:errorcluster)
          }
          frame 1003 {
            w540 = "Dev Error: The Ui.vi for the selected class is broken." ("message")
            n232 = Bundle By Name(cluster=w541, "source"=w540) -> (w539:errorcluster)
          }
          frame 1, 91, 1556, 5001 {
            w544 = "Make sure Variant to data." ("message")
            n233 = Bundle By Name(cluster=w543, "source"=w544) -> (w542:errorcluster)
          }
          frame 15550 {
            n234 = Unbundle By Name(w548) -> ("source"=w550:string)
            n235 = Concatenate Strings(w550, "\n", "*Note : The System does not yet have a configuration to download. Create or open a configuration and download it to the System" ("message")) -> (w546:string)
            n236 = Bundle By Name(cluster=w548, "source"=w546) -> (w545:errorcluster)
          }
          frame -375006, 537549, 538500 {
            n237 = Unbundle By Name(w556) -> ("source"=w552:string)
            n238 = Concatenate Strings(w552, "\n", "*Note : Invalid configuration when opening config file. Check out if it existed or both tags and class names are correct." ("message")) -> (w553:string)
            n239 = Bundle By Name(cluster=w556, "source"=w553) -> (w555:errorcluster)
            n240 = call <vilib>:"Simple Error Handler.vi"("error in (no error)"=w555) -> ()  [unwired: 4 in, 5 out]
          }
          frame 42..44 {
            # "42 : Node Invalid\n43 : Engine unInitialized\n44 : JSON to LVobject"
            n241 = Unbundle By Name(w557) -> ("source"=w558:string)
          }
          frame 402840 {
            # "check out configuration class"
            n242 = Unbundle By Name(w562) -> ("source"=w564:string)
            n243 = Concatenate Strings(w564, "\n", "JSON is blank because identifier unknown to unwrap or wrap " ("message")) -> (w560:string)
            n244 = Bundle By Name(cluster=w562, "source"=w560) -> (w559:errorcluster)
          }
          frame -17006 {
            w565 = "starting application.\nPlease restart LabVIEW program" ("format string")
            # "Teststand UI starting Error"
            n245 = Bundle("Message Name"="Close?", "") -> (w572:cluster{"Message Name":string, string})  [unwired: 1 in]
            n246 = Bundle("notification"="Done", variant) -> (w571:cluster{"notification":string, variant})  [unwired: 1 in]
            n247 = Enqueue Element(queue=w575, element=w572) -> ()  [unwired: 2 in, 3 out]
            n248 = Send Notification(notification=w571, notifier=w568) -> ()  [unwired: 1 in, 2 out]
            n249 = Bundle By Name(cluster=w567, "source"=w565) -> (w566:errorcluster)
          }
        }
        n250 = call "one shot error.vi"("error in"=w505) -> ()  [unwired: 11 in]
        n251 = Format Into String(format string="%1$s\t%2$d\t%3$s\n", w510, w502, w501) -> (resulting string=w517:string)  [unwired: 2 in, 1 out]
        n252 = Not A Number/Path/Refnum?(number/path/refnum=w509) -> (NaN/Path/Refnum?=w508:bool)
        n253 = case shown="True" w508 {
          tunnel: w517 -> [w524 _]
          tunnel: [w523 w525] -> w516
          tunnel: w509 -> [w522 _]
          tunnel: errorcluster {"status"=FALSE, "code"=0, "source"=""} ("error in") -> [w521 w525]
          frame False {
            n254 = Write to Text File(file (use dialog)=w522, text=w524, error in=w521) -> (error out=w523:errorcluster)  [unwired: 1 in, 2 out]
          }
          frame True {
          }
        }
      }
      frame "Missing Message Handler", Default {
        # "Call this case if a message is received that is not handled by any other case. Typically this is a programming error as a result of a typo or unhandled message/missing message handler."
        n255 = property class="VI"(reference=w576) -> (reference out=w577:refnum<vi>, "Name"=w583:string)  [unwired: 1 in, 1 out]
        n256 = Format Into String(format string="DevError: Missing message handler for '%s\" message." ("message"), w581) -> (resulting string=w580:string)  [unwired: 2 in, 1 out]
        n257 = call <vilib>:"Unset Busy.vi"("VI reference (current VI)"=w577) -> ()  [unwired: 10 in, 1 out]
        n258 = call "CEF_error generator.vi"("error in"=w585, "source"=w583, "append error message"=w580, "error code (0)"=538505) -> ("error out"=w578:errorcluster)  [unwired: 5 in]
      }
      frame "Close" {
        w590 = FALSE  # Reset
        n259 = Flatten To String(anything=w590, error in (no error)=w592) -> (data string=w589:string, error out=w591:errorcluster)  [unwired: 2 in, 1 out]
        n260 = Bundle("Control Engines", "data string"=w589) -> (w593:cluster{string, "data string":string})  [unwired: 1 in]
        n261 = Enqueue Element(queue=w595, element=w593, error in (no error)=w591) -> (queue out=w588:refnum<queue>, error out=w596:errorcluster)  [unwired: 1 in, 1 out]
        n262 = Bundle("Write INI File", "") -> (w599:cluster{string, string})  [unwired: 1 in]
        n263 = Enqueue Element(queue=w588, element=w599, error in (no error)=w596) -> (error out=w587:errorcluster)  [unwired: 1 in, 2 out]
        n264 = property class="Pnl"(reference=w600, error in=w587, "DeferPanUpdts"=TRUE ("Defer Panel Updates")) -> (error out=w586:errorcluster)  [unwired: 1 out]
      }
      frame "Write INI File" {
        n265 = Unbundle By Name(w612) -> ("INI file ref"=w603:T6, "paths"=w611:T4)
        n266 = Bundle("Shutdown", "") -> (w610:cluster{string, string})  [unwired: 1 in]
        n267 = Enqueue Element(queue=w604, element=w610, error in (no error)=w606) -> (error out=w605:errorcluster)  [unwired: 1 in, 2 out]
        n268 = call "Write INI File.vi"("error in"=w605, "File path"=w611, "INI refnum"=w603) -> ("error out"=w607:errorcluster)  [unwired: 8 in]
      }
      frame "Shutdown" {
        # "close root DVR"
        n269 = Release Queue(queue=w622, error in (no error)=w623) -> (error out=w619:errorcluster)  [unwired: 1 in, 2 out]
        n270 = property class="Pnl"(reference=w627, "DeferPanUpdts"=FALSE ("Defer Panel Updates")) -> ()  [unwired: 1 in, 2 out]
        n271 = global read "Control Globals.vi" "TestStand Engine"() -> (w620:refnum<k7>)
        n272 = Unbundle By Name(w632) -> ("root"=w630:T2, "Error Log"=w631:refnum<file>, "standard events"=w626:T3)
        n273 = Close Reference(reference=w620, error in (no error)=w619) -> (error out=w618:errorcluster)
        n274 = global read "Control Globals.vi" "Event Callback"() -> (w621:refnum<k27>)
        n275 = Unregister For Events(event registration refnum=w621, error in=w618) -> (error out=w617:errorcluster)
        n276 = call "ClearStandardEvents.vi"("error in"=w617, "standard events"=w626, "sub panel ref in"=w628) -> ("error out"=w624:errorcluster)  [unwired: 8 in]
        n277 = Close File(refnum=w631, error in=w624) -> (error out=w625:errorcluster)  [unwired: 1 out]
        n278 = call "CloseNode.vi"("error in"=w625, "node ref"=w630) -> ("error out"=w615:errorcluster)  [unwired: 9 in]
        n279 = disable-structure shown="RUN_TIME_ENGINE==True" {
          disable-tunnel: w615 -> [w633 w634]
          disable-tunnel: [w633 w634] -> w614
          disable-tunnel: w613 -> [_ _]
          frame condition #0 (active) {
          }
          frame condition #1 {
            n280 = Quit LabVIEW() -> ()  [unwired: 1 in]
          }
        }
      }
      frame "------------Menu Operations--------------" {
        # "Dummy case to add a seperation in the Case Structure menu"
      }
      frame "Close?", "New?", "Open?" {
        n281 = Unbundle By Name(w639) -> ("current path"=w638:path, "unsaved changes"=w640:bool, "repository"=w642:refnum<class "CEF_Repository.lvclass">, "root"=w641:T2)
        n282 = case shown="True" w640 {
          tunnel: w648 -> [w659 w667]
          tunnel: [w659 w660] -> w649
          tunnel: [TRUE ("Cancelled") w662] -> w647
          tunnel: w642 -> [_ w664]
          tunnel: w641 -> [_ w665]
          tunnel: w638 -> [_ w661]
          frame False {
            # "If there is nothing to save Go do Action"
          }
          frame True {
            n283 = call-dynamic "ReadTree.vi"("error in"=w667, "root"=w665, "CEF_Repository in"=w664) -> ("error out"=w666:errorcluster, "CEF_Repository out"=w663:refnum<class "CEF_Repository.lvclass">)  [unwired: 7 in]
            n284 = call "SaveDialog.vi"("error in"=w666, "current path"=w661, "repository"=w663) -> ("error out"=w660:errorcluster, "Done?"=w662:bool)  [unwired: 6 in, 1 out]
          }
        }
        n285 = Search and Replace String(input string=w646, search string="?", replace string="") -> (result string=w637:string)  [unwired: 5 in, 3 out]
        n286 = case shown="True" w647 {
          tunnel: [w651 w656] -> w650
          tunnel: w649 -> [w651 w657]
          tunnel: w643 -> [_ w655]
          tunnel: w637 -> [_ w654]
          frame False {
          }
          frame True {
            n287 = Bundle("result string"=w654, "") -> (w652:cluster{"result string":string, string})  [unwired: 1 in]
            n288 = Enqueue Element(queue=w655, element=w652, error in (no error)=w657) -> (error out=w656:errorcluster)  [unwired: 1 in, 2 out]
          }
        }
      }
      frame "New" {
        n289 = case shown="False" w671 {
          tunnel: w680 -> [w697 _]
          tunnel: w679 -> [w693 w701]
          tunnel: w678 -> [w691 w704]
          tunnel: [w685 w703] -> w676
          tunnel: [w687 path "" ("Configuration file")] -> w672
          tunnel: w683 -> [w694 _]
          tunnel: w670 -> [_ _]
          frame False {
            n290 = Unbundle By Name(w694) -> ("paths.Configuration"=w687:path)
            n291 = Bundle("notification"="Open", "") -> (w692:cluster{"notification":string, string})  [unwired: 1 in]
            n292 = Enqueue Element(queue=w693, element=w692, error in (no error)=w691) -> (error out=w688:errorcluster)  [unwired: 1 in, 2 out]
            n293 = Path To String(path=w687) -> (string=w686:string)
            n294 = Bundle("notification"="Open Config", w686) -> (w695:cluster{"notification":string, string})  [unwired: 1 in]
            n295 = Send Notification(notification=w695, notifier=w697, error in (no error)=w688) -> (error out=w685:errorcluster)  [unwired: 1 out]
          }
          frame True {
            n296 = Bundle("PopulateTree", "") -> (w698:cluster{string, string})  [unwired: 1 in]
            n297 = Enqueue Element(queue=w701, element=w698, error in (no error)=w704) -> (error out=w703:errorcluster)  [unwired: 1 in, 2 out]
          }
        }
        n298 = Unbundle By Name(w683) -> ("paths.Plugin"=w677:path)
        n299 = call-dynamic "Initialize.vi"("error in"=w676, "path"=w677, "CEF_Repository in"=refnum<class "CEF_HierarchyRepo.lvclass"> refnum ("CEF.lvlibp:CEF_HierarchyRepo.lvclass")) -> ("error out"=w681:errorcluster, "CEF_Repository out"=w673:refnum<class "CEF_HierarchyRepo.lvclass">)  [unwired: 7 in]
        n300 = call-dynamic "Initialize.vi"("error in"=w681, "CEF_Serialize node in"=refnum<class "System.lvclass"> refnum ("System.lvlibp:System")) -> ("error out"=w668:errorcluster, "data value reference"=w675:refnum<data-value>)  [unwired: 7 in, 1 out]
        n301 = Bundle By Name(cluster=w683, "unsaved changes"=FALSE, "current path"=w672, "repository"=w673, "root"=w675) -> (w684:T1)
      }
      frame "Open" {
        n302 = Unbundle By Name(w727) -> ("unsaved changes"=w722:bool, "root"=w721:T2, "repository"=w712:refnum<class "CEF_Repository.lvclass">, "current path"=w713:path, "paths.Configuration"=w716:path)
        n303 = case shown="True" w707 {
          tunnel: w706 -> [w728 w730]
          tunnel: [w728 w729] -> w705
          frame False {
          }
          frame True {
            n304 = invoke class="VI" method="FP.Open"(error in=w730) -> (error out=w729:errorcluster)  [unwired: 4 in, 4 out]
          }
        }
        n305 = Equal?(x=w716, y=path "" ("f")) -> (x = y?=w717:bool)
        n306 = Not(x=w717) -> (.not. x?=w719:bool)
        n307 = Not(x=w707) -> (.not. x?=w708:bool)
        n308 = And(x=w719, y=w708) -> (x .and. y?=w710:bool)
        n309 = case shown="False" w710 {
          tunnel: [w733 w734] -> w725
          tunnel: [w732 _] -> w724
          tunnel: w716 -> [w731 w734]
          frame False {
            n310 = call "FileDialog.vi"("start path"=w731) -> ("cancelled"=w732:bool, "selected path"=w733:path)  [unwired: 8 in, 1 out]
          }
          frame True {
          }
        }
        n311 = case shown="False" w724 {
          tunnel: [w736 w769] -> w711
          tunnel: w705 -> [w749 w769]
          tunnel: w721 -> [w744 w770]
          tunnel: [w742 w771] -> w715
          tunnel: w725 -> [w745 w771]
          tunnel: w722 -> [_ w772]
          tunnel: [FALSE ("unsaved changes") w772] -> w723
          tunnel: [w743 w770] -> w720
          tunnel: w713 -> [w741 _]
          tunnel: w712 -> [w739 w768]
          tunnel: [w740 w768] -> w714
          tunnel: w708 -> [w738 _]
          tunnel: w709 -> [w737 _]
          frame False {
            n312 = call-dynamic "Open.vi"("error in"=w749, "file path"=w745, "CEF_Repository in"=w739) -> ("error out"=w747:errorcluster, "invalid?"=w748:bool, "CEF_Repository out"=w746:refnum<class "CEF_Repository.lvclass">)  [unwired: 6 in]
            n313 = case shown="False" w748 {
              tunnel: [w760 w767] -> w740
              tunnel: [w751 w763] -> w736
              tunnel: [w757 w766] -> w743
              tunnel: w746 -> [w759 w767]
              tunnel: w747 -> [w756 w763]
              tunnel: w745 -> [w758 _]
              tunnel: w744 -> [_ w766]
              tunnel: [w758 w765] -> w742
              tunnel: w741 -> [_ w765]
              tunnel: w738 -> [w754 _]
              tunnel: [w752 w761] -> w735
              frame False {
                n314 = call-dynamic "WriteTree.vi"("error in"=w756, "CEF_Repository in"=w759) -> ("error out"=w751:errorcluster, "root"=w757:refnum<data-value>, "CEF_Repository out"=w760:refnum<class "CEF_Repository.lvclass">)  [unwired: 7 in]
                n315 = Flatten To String(anything=w754) -> (data string=w753:string)  [unwired: 3 in, 2 out]
                n316 = Bundle("Control Engines", "data string"=w753) -> (w752:cluster{string, "data string":string})  [unwired: 1 in]
              }
              frame True {
                n317 = Bundle("notification"="PopulateTree", "") -> (w761:cluster{"notification":string, string})  [unwired: 1 in]
              }
            }
            n318 = Enqueue Element(queue=w737, element=w735) -> ()  [unwired: 2 in, 3 out]
          }
          frame True {
          }
        }
        n319 = Bundle By Name(cluster=w727, "unsaved changes"=w723, "root"=w720, "repository"=w714, "current path"=w715, "paths.Configuration"=w715) -> (w726:T1)
      }
      frame "Save" {
        n320 = Unbundle By Name(w782) -> ("current path"=w783:path, "repository"=w773:refnum<class "CEF_Repository.lvclass">, "root"=w784:T2)
        n321 = Empty String/Path?(string/path=w783) -> (empty?=w785:bool)
        n322 = Not A Number/Path/Refnum?(number/path/refnum=w783) -> (NaN/Path/Refnum?=w786:bool)
        n323 = call-dynamic "ReadTree.vi"("error in"=w774, "root"=w784, "CEF_Repository in"=w773) -> ("error out"=w780:errorcluster, "CEF_Repository out"=w779:refnum<class "CEF_Repository.lvclass">)  [unwired: 7 in]
        n324 = Or(x=w785, y=w786) -> (x .or. y?=w787:bool)
        n325 = case shown="True" w787 {
          tunnel: w783 -> [w790 w800]
          tunnel: [w790 w799] -> w775
          tunnel: w780 -> [w792 w794]
          tunnel: w779 -> [w791 w797]
          tunnel: [w788 w796] -> w778
          tunnel: [w789 w795] -> w777
          frame False {
            # "unchanged file path"
            n326 = call-dynamic "Save.vi"("error in"=w792, "file path"=w790, "CEF_Repository in"=w791) -> ("error out"=w789:errorcluster, "CEF_Repository out"=w788:refnum<class "CEF_Repository.lvclass">)  [unwired: 7 in]
          }
          frame True {
            # "Empthy path, Not a Path, and changed"
            n327 = call "FileDialog.vi"("error in"=w794, "start path"=w800) -> ("error out"=w793:errorcluster, "cancelled"=w801:bool, "selected path"=w798:path)  [unwired: 7 in]
            n328 = case shown="False" w801 {
              tunnel: [w804 w809] -> w799
              tunnel: w798 -> [w804 w809]
              tunnel: w793 -> [w806 w807]
              tunnel: w797 -> [w805 w808]
              tunnel: [w803 w808] -> w796
              tunnel: [w802 w807] -> w795
              frame False {
                n329 = call-dynamic "Save.vi"("error in"=w806, "file path"=w804, "CEF_Repository in"=w805) -> ("error out"=w802:errorcluster, "CEF_Repository out"=w803:refnum<class "CEF_Repository.lvclass">)  [unwired: 7 in]
              }
              frame True {
              }
            }
          }
        }
        n330 = Unbundle By Name(w777) -> ("status"=w776:bool)
        n331 = Bundle By Name(cluster=w782, "paths.Configuration"=w775, "current path"=w775, "repository"=w778, "unsaved changes"=w776) -> (w781:T1)
      }
      frame "SaveAs" {
        n332 = Unbundle By Name(w816) -> ("current path"=w817:path, "repository"=w811:refnum<class "CEF_Repository.lvclass">, "root"=w822:T2)
        n333 = call-dynamic "ReadTree.vi"("error in"=w812, "root"=w822, "CEF_Repository in"=w811) -> ("error out"=w819:errorcluster, "CEF_Repository out"=w818:refnum<class "CEF_Repository.lvclass">)  [unwired: 7 in]
        n334 = call "FileDialog.vi"("error in"=w819, "start path"=w817) -> ("error out"=w820:errorcluster, "cancelled"=w821:bool, "selected path"=w810:path)  [unwired: 7 in]
        n335 = case shown="False" w821 {
          tunnel: w810 -> [w825 _]
          tunnel: w820 -> [w827 w828]
          tunnel: w818 -> [w826 w829]
          tunnel: [w824 w829] -> w815
          tunnel: [w823 w828] -> w814
          frame False {
            n336 = call-dynamic "Save.vi"("error in"=w827, "file path"=w825, "CEF_Repository in"=w826) -> ("error out"=w823:errorcluster, "CEF_Repository out"=w824:refnum<class "CEF_Repository.lvclass">)  [unwired: 7 in]
          }
          frame True {
          }
        }
        n337 = Bundle By Name(cluster=w816, "paths.Configuration"=w810, "current path"=w810, "repository"=w815) -> (w813:T1)
      }
      frame "-------TreeControl Operations-----------" {
        # "Dummy case to add a seperation in the Case Structure menu"
      }
      frame "AddNode" {
        n338 = Unbundle By Name(w860) -> ("glyph manager"=w859:T5, "repository"=w846:refnum<class "CEF_Repository.lvclass">)
        n339 = Unflatten From String(type=T8 {"subNode"="", "Node ID"=""} ("input cluster"), binary string=w852, error in (no error)=w853) -> (value=w854:T8, error out=w848:errorcluster)  [unwired: 2 in, 1 out]
        n340 = Unbundle By Name(w854) -> ("Node ID"=w851:string, "subNode"=w842:string)
        n341 = call-dynamic "GetClassPath.vi"("error in"=w848, "class name"=w842, "CEF_Repository in"=w846) -> ("error out"=w844:errorcluster, "class path"=w847:path)  [unwired: 6 in, 1 out]
        n342 = call <vilib>:"Get LV Class Default Value.vi"("error in (no error)"=w844, "class path"=w847) -> ("error out"=w843:errorcluster, "object"=w845:refnum<class>)  [unwired: 8 in]
        n343 = To More Specific Class(target class=refnum<class "CEF_serializable node.lvclass"> refnum ("CEF.lvlibp:CEF_serializable node.lvclass"), reference=w845, error in=w843) -> (specific class reference=w849:refnum<class "CEF_serializable node.lvclass">, error out=w850:errorcluster)
        n344 = call "AddNode.vi"("error in"=w850, "parameters"=w842, "parent node ID"=w851, "CEF_Node in"=w849) -> ("error out"=w858:errorcluster, "summary"=w840:T18)  [unwired: 6 in]
        n345 = call "PopulateTreeSumaryWithGlyphManager.vi"("error in"=w858, "glyph manager"=w859, "summary"=w840, "tree ref in"=w832) -> ("error out"=w839:errorcluster, "glyph manager out"=w856:T17)  [unwired: 6 in]
        n346 = Index Array(array=w840) -> (element=w841:T19)  [unwired: 1 in]
        n347 = Unbundle By Name(w841) -> ("ID"=w835:string)
        n348 = Bundle By Name(cluster=w860, "unsaved changes"=TRUE, "glyph manager"=w856) -> (w861:T1)
        n349 = Bundle("format string"="RefreshNode", "ID"=w835) -> (w833:cluster{"format string":string, "ID":string})  [unwired: 1 in]
        n350 = Enqueue Element(queue=w834, element=w833, error in (no error)=w839) -> (error out=w838:errorcluster)  [unwired: 1 in, 2 out]
      }
      frame "Duplicate" {
        n351 = Unbundle By Name(w869) -> ("glyph manager"=w866:T5)
        n352 = call "IDtoNode.vi"("error in"=w863, "ID"=w864) -> ("error out"=w871:errorcluster, "invalid Id"=w870:bool, "node ref"=w872:refnum<data-value>)  [unwired: 7 in]
        n353 = case shown="False" w870 {
          tunnel: [w884 w886] -> w873
          tunnel: w872 -> [w883 _]
          tunnel: w871 -> [w880 w887]
          tunnel: w866 -> [w876 w890]
          tunnel: [w875 w890] -> w865
          tunnel: w862 -> [w874 _]
          frame False {
            n354 = call "DuplicateNode.vi"("same parent?"=TRUE ("s"), "error in"=w880, "node ref in"=w883) -> ("error out"=w881:errorcluster, "new node ref"=w882:refnum<data-value>)  [unwired: 7 in]
            n355 = call "Summary.vi"("error in"=w881, "node self ref"=w882) -> ("error out"=w878:errorcluster, "summary"=w877:T18)  [unwired: 8 in]
            n356 = call "PopulateTreeSumaryWithGlyphManager.vi"("error in"=w878, "glyph manager"=w876, "summary"=w877, "tree ref in"=w874) -> ("error out"=w884:errorcluster, "glyph manager out"=w875:T17)  [unwired: 6 in]
          }
          frame True {
            n357 = call "CEF_error generator.vi"("error in"=w887, "source"="TSS::Duplicate", "append error message"="Node invalid " ("source"), "error code (0)"=42) -> ("error out"=w886:errorcluster)  [unwired: 5 in]
          }
        }
        n358 = Bundle By Name(cluster=w869, "unsaved changes"=TRUE, "glyph manager"=w865) -> (w868:T1)
      }
      frame "CustomMenuAction" {
        n359 = Unbundle By Name(w898) -> ("standard events.node change"=w895:refnum<user-event>)
        n360 = Match Pattern(string=w899, regular expression=":") -> (before substring=w902:string, after substring=w896:string)  [unwired: 1 in, 2 out]
        n361 = call "IDtoNode.vi"("error in"=w893, "ID"=w896) -> ("error out"=w892:errorcluster, "invalid Id"=w903:bool, "node ref"=w904:refnum<data-value>)  [unwired: 7 in]
        n362 = case shown="False" w903 {
          tunnel: [w916 w950] -> w900
          tunnel: w904 -> [w914 _]
          tunnel: w892 -> [w910 w951]
          tunnel: w902 -> [w917 _]
          tunnel: w894 -> [w915 _]
          tunnel: w897 -> [w912 _]
          tunnel: w895 -> [w908 _]
          tunnel: w891 -> [w905 _]
          frame False {
            n363 = in-place {
              in-place-border: [w947] -> w918
              in-place-border: w917 -> [w943]
              in-place-border: w915 -> [w946]
              in-place-border: [w945] -> w913
              in-place-border: w912 -> [w939]
              in-place-border: [w943] -> w911
              in-place-border: w910 -> [w942]
              in-place-border: [w941] -> w909
              in-place-border: w908 -> [w940]
              in-place-border: [w940] -> w907
              in-place-border: w905 -> [w938]
              n364 = in-place-dvr #5(w914) -> (w944:refnum<class "CEF_Node.lvclass">)  [unwired: 1 out]
              n365 = call-dynamic "MenuHandler.vi"("tree control"=w946, "main queue"=w939, "error in"=w942, "parameters"=w938, "menu string"=w943, "CEF_Node in"=w944) -> ("error out"=w941:errorcluster, "refresh tree?"=w945:bool, "Unhandled"=w947:bool, "CEF_Node out"=w948:refnum<class "CEF_Node.lvclass">)  [unwired: 2 in]
              n366 = in-place-dvr #5(w948) -> (w906:refnum<data-value>)  [unwired: 1 out]
            }
            n367 = case shown="False" w918 {
              tunnel: w911 -> [_ w929]
              tunnel: [w923 w930] -> w916
              tunnel: w909 -> [w921 w931]
              tunnel: w913 -> [w922 _]
              tunnel: w907 -> [w920 _]
              tunnel: w906 -> [w919 _]
              frame False {
                n368 = case shown="True" w922 {
                  tunnel: [w924 w925] -> w923
                  tunnel: w921 -> [w924 w926]
                  tunnel: w920 -> [_ w928]
                  tunnel: w919 -> [_ w927]
                  frame False {
                  }
                  frame True {
                    # "update EngineMap"
                    n369 = Generate User Event(user event=w928, event data cluster=w927, error in=w926) -> (error out=w925:errorcluster)  [unwired: 1 in, 1 out]
                  }
                }
              }
              frame True {
                n370 = disable-structure shown="Default" {
                  disable-tunnel: w931 -> [w934 w937]
                  disable-tunnel: [w933 w937] -> w930
                  disable-tunnel: w929 -> [w932 _]
                  frame condition #0 {
                    n371 = call "CEF_error generator.vi"("error in"=w934, "source"="TSS::CustomMenuAction", "append error message"=w932, "error code (0)"=538506) -> ("error out"=w933:errorcluster)  [unwired: 5 in]
                  }
                  frame condition #1 (active) {
                  }
                }
              }
            }
          }
          frame True {
            n372 = call "CEF_error generator.vi"("error in"=w951, "source"="TSS:CustomMenuAction", "append error message"="Node invalid " ("source"), "error code (0)"=42) -> ("error out"=w950:errorcluster)  [unwired: 5 in]
          }
        }
      }
      frame "RefreshNode" {
        # "Refreshes the node in the Tree, Sets the save flag to true. This case can be called from the UIs of the nodes"
        n373 = Unbundle By Name(w968) -> ("glyph manager"=w959:T5, "root"=w955:T2)
        n374 = call "IDtoNode.vi"("error in"=w970, "ID"=w961) -> ("error out"=w960:errorcluster, "invalid Id"=w964:bool, "node ref"=w963:refnum<data-value>)  [unwired: 7 in]
        n375 = Select(t=w955, s=w964, f=w963) -> (s? t:f=w962:T2)
        n376 = call "SummaryWithGlyphManager.vi"("error in"=w960, "glyph manager"=w959, "node self ref"=w962) -> ("error out"=w958:errorcluster, "glyph manager out"=w965:T17, "summary"=w957:T18)  [unwired: 6 in]
        n377 = call "RefreshSubTreeWithGlyphManager.vi"("error in"=w958, "glyph manager"=w965, "node information"=w957, "tree ref in"=w954) -> ("error out"=w967:errorcluster, "glyph manager out"=w969:T17, "tree ref out"=w966:refnum<vi>)  [unwired: 5 in]
        n378 = Close Reference(reference=w966, error in (no error)=w967) -> (error out=w956:errorcluster)
        n379 = Bundle By Name(cluster=w968, "glyph manager"=w969) -> (w971:T1)
      }
      frame "RemoveNode" {
        n380 = call "IDtoNode.vi"("error in"=w981, "ID"=w977) -> ("error out"=w980:errorcluster, "invalid Id"=w978:bool, "node ref"=w979:refnum<data-value>)  [unwired: 7 in]
        n381 = case shown="False" w978 {
          tunnel: w980 -> [w983 w990]
          tunnel: w979 -> [w984 _]
          tunnel: [w985 w989] -> w974
          tunnel: w972 -> [w982 _]
          frame False {
            n382 = call "RemoveNode.vi"("error in"=w983, "node"=w984) -> ("error out"=w986:errorcluster, "node ID"=w987:string)  [unwired: 8 in]
            n383 = call "ClearTreeNode.vi"("error in"=w986, "tag"=w987, "tree reference"=w982) -> ("error out"=w985:errorcluster)  [unwired: 8 in]
          }
          frame True {
            n384 = call "CEF_error generator.vi"("error in"=w990, "source"="TSS:RemoveNode", "append error message"="Node invalid " ("source"), "error code (0)"=42) -> ("error out"=w989:errorcluster)  [unwired: 5 in]
          }
        }
        n385 = Bundle By Name(cluster=w973, "unsaved changes"=TRUE) -> (w975:T1)
      }
      frame "PopulateTree" {
        # "Close the Launch Panel, and show the main UI panel"
        n386 = call <vilib>:"Set Busy.vi"("error in (no error)"=w1008) -> ("error out"=w998:errorcluster)  [unwired: 9 in, 1 out]
        n387 = case shown="False" w1000 {
          tunnel: w999 -> [w1020 _]
          tunnel: w998 -> [w1017 w1021]
          tunnel: [w1016 w1021] -> w997
          frame False {
            n388 = Bundle("notification"="Launched", "") -> (w1018:cluster{"notification":string, string})  [unwired: 1 in]
            n389 = Send Notification(notification=w1018, notifier=w1020, error in (no error)=w1017) -> (error out=w1016:errorcluster)  [unwired: 1 out]
          }
          frame True {
          }
        }
        n390 = Unbundle By Name(w1014) -> ("root"=w1005:T2, "glyph manager"=w1002:T5, "standard events.user event"=w1009:refnum<user-event>)
        n391 = call "ClearSubPanel.vi"("error in"=w997, "user event ref"=w1009, "sub panel ref in"=w1003) -> ("error out"=w1006:errorcluster)  [unwired: 7 in, 1 out]
        n392 = call "SummaryWithGlyphManager.vi"("error in"=w1006, "glyph manager"=w1002, "node self ref"=w1005) -> ("error out"=w993:errorcluster, "glyph manager out"=w1007:T17, "summary"=w994:T18)  [unwired: 6 in]
        n393 = case shown="\"\"" w1011 {
          selector: w1011 -> [w1022 _]
          tunnel: w994 -> [_ w1024]
          tunnel: [w1022 w1023] -> w1010
          frame Default {
          }
          frame "" {
            n394 = Index Array(array=w1024) -> (element=w1025:T19)  [unwired: 1 in]
            n395 = Unbundle By Name(w1025) -> ("ID"=w1023:string)
          }
        }
        n396 = property class="Tree (strict)"(reference=w1004, "Val(Sgnl)"=w1010) -> (reference out=w996:refnum<vi>)  [unwired: 1 in, 1 out]
        n397 = call "RefreshEntireTreeWithGlyphManager.vi"("calling VI"=w1001, "error in"=w993, "glyph manager"=w1007, "array"=w994, "tree ref in"=w996) -> ("error out"=w995:errorcluster, "glyph manager out"=w1012:T17)  [unwired: 5 in]
        n398 = Bundle By Name(cluster=w1014, "glyph manager"=w1012) -> (w1013:T1)
      }
      frame "ActivateNode" {
        n399 = Unbundle By Name(w1037) -> ("standard events"=w1031:T3)
        n400 = property class="Pnl"(reference=w1026, "DeferPanUpdts"=TRUE ("Defer Panel Updates")) -> (reference out=w1029:refnum<vi>)  [unwired: 1 in, 1 out]
        n401 = call "IDtoNode.vi"("error in"=w1028, "ID"=w1030) -> ("error out"=w1035:errorcluster, "invalid Id"=w1038:bool, "node ref"=w1036:refnum<data-value>)  [unwired: 7 in]
        n402 = case shown="False" w1038 {
          tunnel: w1036 -> [w1049 _]
          tunnel: [w1043 w1054] -> w1033
          tunnel: w1035 -> [w1041 w1055]
          tunnel: w1031 -> [w1039 _]
          tunnel: w1027 -> [w1047 _]
          tunnel: w1034 -> [w1045 _]
          tunnel: w1029 -> [w1048 _]
          tunnel: w1030 -> [_ w1052]
          frame False {
            n403 = Unbundle By Name(w1039) -> ("user event"=w1046:refnum<user-event>)
            n404 = call "ClearSubPanel.vi"("error in"=w1041, "user event ref"=w1046, "sub panel ref in"=w1047) -> ("error out"=w1040:errorcluster)  [unwired: 7 in, 1 out]
            n405 = call "LoadNodeUIStandardEvents.vi"("Standard Event"=w1039, "error in"=w1040, "sub panel ref"=w1047, "main queue"=w1045, "node"=w1049) -> ("error out"=w1044:errorcluster)  [unwired: 6 in]
            n406 = property class="Pnl"(reference=w1048, error in=w1044, "DeferPanUpdts"=FALSE ("Defer Panel Updates")) -> (error out=w1043:errorcluster)  [unwired: 1 out]
          }
          frame True {
            n407 = Format Into String(format string="%s node is invalid" ("initial string"), w1052) -> (resulting string=w1050:string)  [unwired: 2 in, 1 out]
            n408 = call "CEF_error generator.vi"("error in"=w1055, "source"="TSS::ActivateNode", "append error message"=w1050, "error code (0)"=42) -> ("error out"=w1054:errorcluster)  [unwired: 5 in]
          }
        }
      }
      frame "Move" {
        n409 = Unflatten From String(type=T9 {"node ref"=refnum, "new parent"=refnum, "Index"=0} ("Cluster"), binary string=w1075, error in (no error)=w1072) -> (value=w1073:T9, error out=w1068:errorcluster)  [unwired: 2 in, 1 out]
        n410 = Unbundle By Name(w1073) -> ("Index"=w1057:i32, "node ref"=w1064:T2, "new parent"=w1076:T2)
        n411 = call "MoveNode.vi"("error in"=w1068, "index"=w1057, "new parent"=w1076, "node"=w1064) -> ("error out"=w1066:errorcluster)  [unwired: 7 in]
        n412 = call "Summary.vi"("error in"=w1066, "node self ref"=w1064) -> ("error out"=w1065:errorcluster, "summary"=w1062:T18)  [unwired: 8 in]
        n413 = Index Array(array=w1062, index=w1057) -> (element=w1063:T19)
        n414 = Unbundle By Name(w1063) -> ("ID"=w1060:string)
        n415 = Bundle By Name(cluster=w1069, "unsaved changes"=TRUE) -> (w1070:T1)
        n416 = Bundle("PopulateTree", "ID"=w1060) -> (w1058:cluster{string, "ID":string})  [unwired: 1 in]
        n417 = Enqueue Element(queue=w1059, element=w1058, error in (no error)=w1065) -> (error out=w1067:errorcluster)  [unwired: 1 in, 2 out]
      }
      frame "NodeDataChange" {
        n418 = Unbundle By Name(w1092) -> ("root"=w1079:T2)
        n419 = property class="NISE_CEF_Node"(reference=w1079) -> ("DataAccess:Children"=w1080:refnum<data-value>[])  [unwired: 1 in, 2 out]
        n420 = Index Array(array=w1080) -> (element=w1078:refnum<data-value>)  [unwired: 1 in]
        n421 = call "Find Engine from Child.vi"("error in (no error)"=w1090, "Node ID"=w1091, "HW Engine"=w1078) -> ("error out"=w1084:errorcluster, "Engine"=w1089:refnum<data-value>)  [unwired: 7 in]
        n422 = in-place {
          in-place-border: w1081 -> [w1101]
          in-place-border: w1085 -> [w1098]
          in-place-border: w1084 -> [w1100]
          in-place-border: [w1099] -> w1083
          in-place-border: [w1098] -> w1082
          in-place-border: w1077 -> [w1096]
          n423 = in-place-dvr #6(w1089) -> (w1102:refnum<class "CEF_Node.lvclass">)  [unwired: 1 out]
          n424 = call-dynamic "MenuHandler.vi"("tree control"=w1101, "main queue"=w1098, "error in"=w1100, "parameters"=w1096, "menu string"="Reset Engine" ("message value"), "CEF_Node in"=w1102) -> ("error out"=w1099:errorcluster, "CEF_Node out"=w1103:refnum<class "CEF_Node.lvclass">)  [unwired: 2 in, 2 out]
          n425 = in-place-dvr #6(w1103) -> ()  [unwired: 2 out]
        }
        n426 = Bundle By Name(cluster=w1092, "unsaved changes"=TRUE) -> (w1095:T1)
        n427 = Bundle("message name"="RefreshNode", "") -> (w1086:cluster{"message name":string, string})  [unwired: 1 in]
        n428 = Enqueue Element(queue=w1082, element=w1086, error in (no error)=w1083) -> (error out=w1093:errorcluster)  [unwired: 1 in, 2 out]
      }
      frame "-------Engine Operations-----------" {
      }
      frame "Export Engine" {
        n429 = Unbundle By Name(w1109) -> ("repository"=w1111:refnum<class "CEF_Repository.lvclass">, "current path"=w1106:path)
        n430 = call "IDtoNode.vi"("error in"=w1116, "ID"=w1115) -> ("error out"=w1112:errorcluster, "invalid Id"=w1114:bool, "node ref"=w1113:refnum<data-value>)  [unwired: 7 in]
        n431 = case shown="False" w1114 {
          tunnel: w1113 -> [w1121 _]
          tunnel: w1112 -> [w1118 w1143]
          tunnel: w1111 -> [w1126 w1140]
          tunnel: [w1124 w1142] -> w1110
          tunnel: [w1123 w1140] -> w1107
          tunnel: w1106 -> [w1122 _]
          frame False {
            n432 = property class="NISE_CEF_Node"(reference=w1121, error in=w1118) -> (reference out=w1119:refnum<data-value>, error out=w1117:errorcluster, "DataAccess:NodeClass"=w1120:string)
            n433 = call "FileDialog.vi"("error in"=w1117, "default name"=w1120, "start path"=w1122) -> ("error out"=w1127:errorcluster, "cancelled"=w1128:bool, "selected path"=w1125:path)  [unwired: 6 in]
            n434 = case shown="False" w1128 {
              tunnel: w1127 -> [w1136 w1137]
              tunnel: w1119 -> [w1135 _]
              tunnel: w1126 -> [w1134 w1138]
              tunnel: w1125 -> [w1129 _]
              tunnel: [w1131 w1137] -> w1124
              tunnel: [w1130 w1138] -> w1123
              frame False {
                n435 = call-dynamic "ReadTree.vi"("error in"=w1136, "root"=w1135, "CEF_Repository in"=w1134) -> ("error out"=w1132:errorcluster, "CEF_Repository out"=w1133:refnum<class "CEF_Repository.lvclass">)  [unwired: 7 in]
                n436 = call-dynamic "Save.vi"("error in"=w1132, "file path"=w1129, "CEF_Repository in"=w1133) -> ("error out"=w1131:errorcluster, "CEF_Repository out"=w1130:refnum<class "CEF_Repository.lvclass">)  [unwired: 7 in]
              }
              frame True {
              }
            }
          }
          frame True {
            n437 = call "CEF_error generator.vi"("error in"=w1143, "source"="TSS::Export Engine", "append error message"="Invalid Node" ("source"), "error code (0)"=42) -> ("error out"=w1142:errorcluster)  [unwired: 5 in]
          }
        }
        n438 = Bundle By Name(cluster=w1109, "repository"=w1107) -> (w1108:T1)
      }
      frame "Import Engine" {
        n439 = Unbundle By Name(w1156) -> ("root"=w1147:T2, "repository"=w1159:refnum<class "CEF_Repository.lvclass">, "current path"=w1152:path)
        n440 = call "IDtoNode.vi"("error in"=w1151, "ID"=w1146) -> ("error out"=w1150:errorcluster, "node ref"=w1149:refnum<data-value>)  [unwired: 7 in, 1 out]
        n441 = call "FileDialog.vi"("error in"=w1150, "start path"=w1152) -> ("error out"=w1160:errorcluster, "cancelled"=w1153:bool, "selected path"=w1157:path)  [unwired: 7 in]
        n442 = case shown="True" w1153 {
          tunnel: w1160 -> [w1171 w1203]
          tunnel: w1159 -> [w1170 w1202]
          tunnel: w1158 -> [w1167 _]
          tunnel: w1157 -> [w1163 _]
          tunnel: [w1166 w1201] -> w1148
          tunnel: [w1165 w1202] -> w1145
          tunnel: [w1164 w1203] -> w1154
          tunnel: w1149 -> [w1162 _]
          tunnel: w1147 -> [w1161 w1201]
          frame False {
            n443 = call-dynamic "Open.vi"("error in"=w1171, "file path"=w1163, "CEF_Repository in"=w1170) -> ("error out"=w1168:errorcluster, "invalid?"=w1172:bool, "CEF_Repository out"=w1169:refnum<class "CEF_Repository.lvclass">)  [unwired: 6 in]
            n444 = case shown="False" w1172 {
              tunnel: [w1190 w1191] -> w1165
              tunnel: [w1187 w1199] -> w1164
              tunnel: [w1178 w1194] -> w1166
              tunnel: w1169 -> [w1188 w1191]
              tunnel: w1168 -> [w1189 w1200]
              tunnel: w1167 -> [w1173 _]
              tunnel: w1163 -> [_ w1196]
              tunnel: w1162 -> [w1186 _]
              tunnel: w1161 -> [w1183 w1194]
              frame False {
                n445 = call-dynamic "WriteTree.vi"("error in"=w1189, "CEF_Repository in"=w1188) -> ("error out"=w1184:errorcluster, "root"=w1185:refnum<data-value>, "CEF_Repository out"=w1190:refnum<class "CEF_Repository.lvclass">)  [unwired: 7 in]
                n446 = call "LinkNodes.vi"("error in"=w1184, "child in"=w1185, "parent in"=w1186) -> ("error out"=w1182:errorcluster, "parent out"=w1180:refnum<data-value>)  [unwired: 6 in, 1 out]
                n447 = call "LinkNodes.vi"("error in"=w1182, "child in"=w1180, "parent in"=w1183) -> ("error out"=w1181:errorcluster, "parent out"=w1179:refnum<data-value>)  [unwired: 6 in, 1 out]
                n448 = Bundle("PopulateTree", "") -> (w1174:cluster{string, string})  [unwired: 1 in]
                n449 = call "UnlinkNode.vi"("error in"=w1181, "child in"=w1180, "parent in"=w1179) -> ("error out"=w1177:errorcluster, "parent out"=w1178:refnum<data-value>)  [unwired: 6 in, 1 out]
                n450 = Enqueue Element(queue=w1173, element=w1174, error in (no error)=w1177) -> (error out=w1187:errorcluster)  [unwired: 1 in, 2 out]
              }
              frame True {
                n451 = Strip Path(path=w1196) -> (name=w1195:string)  [unwired: 1 out]
                n452 = Format Into String(format string="%s config invalid " ("source"), w1195) -> (resulting string=w1193:string)  [unwired: 2 in, 1 out]
                n453 = call "CEF_error generator.vi"("error in"=w1200, "source"="TSS::Import Engine", "append error message"=w1193, "error code (0)"=42) -> ("error out"=w1199:errorcluster)  [unwired: 5 in]
              }
            }
          }
          frame True {
          }
        }
        n454 = Bundle By Name(cluster=w1156, "repository"=w1145, "root"=w1148) -> (w1155:T1)
      }
      frame "Control Engines" {
        # "Engines"
        # "0 : HW Engine\n1 : Special Test"
        n455 = Unbundle By Name(w1222) -> ("root"=w1223:T2)
        n456 = Unflatten From String(type=TRUE, binary string=w1215, error in (no error)=w1216) -> (value=w1213:bool, error out=w1209:errorcluster)  [unwired: 2 in, 1 out]
        n457 = property class="NISE_CEF_Node"(reference=w1223) -> ("DataAccess:Children"=w1221:refnum<data-value>[])  [unwired: 1 in, 2 out]
        n458 = Index Array(array=w1221) -> (element=w1220:refnum<data-value>)  [unwired: 1 in]
        n459 = Bundle("PopulateTree", "") -> (w1212:cluster{string, string})  [unwired: 1 in]
        n460 = property class="NISE_CEF_Node"(reference=w1220) -> ("DataAccess:Children"=w1219:refnum<data-value>[])  [unwired: 1 in, 2 out]
        n461 = Enqueue Element(queue=w1207, element=w1212, error in (no error)=w1209) -> (error out=w1208:errorcluster)  [unwired: 1 in, 2 out]
        n462 = for {
          tunnel: w1219 -> [w1230] mode=indexing
          shift-right: [w1233] -> w1206
          shift-left: w1208 -> [w1229]
          tunnel: w1218 -> [w1231]
          tunnel: w1217 -> [w1228]
          tunnel: w1207 -> [w1232]
          tunnel: w1213 -> [w1227]
          n463 = in-place {
            in-place-border: w1229 -> [w1234]
            in-place-border: [w1239] -> w1233
            in-place-border: w1232 -> [w1237]
            in-place-border: w1231 -> [w1241]
            in-place-border: w1228 -> [w1238]
            in-place-border: w1227 -> [w1235]
            n464 = in-place-dvr #7(w1230) -> (w1242:refnum<class "CEF_Node.lvclass">)  [unwired: 1 out]
            n465 = case shown="True" w1235 {
              tunnel: ["Reset Engine" ("message value") "Initialize Engine" ("message value")] -> w1236
              frame False {
              }
              frame True {
                n466 = Wait (ms)(milliseconds to wait=u32 300) -> ()  [unwired: 1 out]
              }
            }
            n467 = call-dynamic "MenuHandler.vi"("tree control"=w1241, "main queue"=w1237, "error in"=w1234, "parameters"=w1238, "menu string"=w1236, "CEF_Node in"=w1242) -> ("error out"=w1239:errorcluster, "CEF_Node out"=w1240:refnum<class "CEF_Node.lvclass">)  [unwired: 2 in, 2 out]
            n468 = in-place-dvr #7(w1240) -> ()  [unwired: 2 out]
          }
        }
        n469 = case shown="False" w1205 {
          tunnel: w1206 -> [w1225 w1226]
          tunnel: [w1224 w1226] -> w1204
          frame False {
            n470 = invoke class="VI" method="FP.Open"(error in=w1225) -> (error out=w1224:errorcluster)  [unwired: 4 in, 4 out]
          }
          frame True {
          }
        }
      }
      frame "Record Engines" {
        n471 = Unflatten From String(type=TRUE, binary string=w1253, error in (no error)=w1254) -> (value=w1252:bool, error out=w1251:errorcluster)  [unwired: 2 in, 1 out]
        n472 = case shown="False" w1252 {
          selector: w1252 -> [_ w1275]
          tunnel: w1251 -> [w1262 w1267]
          tunnel: [w1258 w1273] -> w1250
          tunnel: w1249 -> [w1261 w1277]
          tunnel: [w1260 w1276] -> w1248
          tunnel: w1247 -> [_ _]
          tunnel: w1246 -> [_ _]
          frame False {
            n473 = Unbundle By Name(w1261) -> ("tdms file"=w1257:refnum<k34>)
            n474 = TDMS Close(8:w1262, 11:w1257) -> (0:w1258:errorcluster)  [unwired: 1 out]
            n475 = Bundle By Name(cluster=w1261, "tdms file"=refnum<k34> refnum, "Record"=FALSE) -> (w1260:T1)
          }
          frame True {
            n476 = Unbundle By Name(w1277) -> ("paths.Data"=w1270:path)
            n477 = Get Date/Time In Seconds() -> (seconds since 1Jan1904=w1271:timestamp)
            n478 = Format Into String(format string="%<%Y%m%d_%H%M%S>T.tdms", w1271) -> (resulting string=w1269:string)  [unwired: 2 in, 1 out]
            n479 = Build Path(base path=w1270, name or relative path=w1269) -> (appended path=w1268:path)
            n480 = TDMS Open(5:FALSE ("create index file? (T)"), 8:w1267, 10:T16."open or create" ("operation (0:open)"), 11:w1268) -> (0:w1266:errorcluster, 3:w1263:refnum<k34>)  [unwired: 3 in]
            n481 = case shown="Error .." w1266 {
              selector: w1266 -> [w1279 w1286]
              tunnel: [w1283 w1286] -> w1273
              tunnel: w1275 -> [_ w1288]
              tunnel: [TRUE ("Record") FALSE ("Record")] -> w1274
              frame No Error {
                n482 = property on="Time" class="DigNum (strict)"(error in=w1279, "Value"=0.0 ("Time")) -> (error out=w1278:errorcluster)  [unwired: 1 in, 1 out]
                n483 = call "Timing FGV.vi"("Time Target (s)"=5, "Timer Mode"=T15."Start Timer", "Error In"=w1278) -> ("Error Out"=w1283:errorcluster)  [unwired: 6 in, 2 out]
              }
              frame Error {
                n484 = Not(x=w1288) -> (.not. x?=w1287:bool)
                n485 = property on="Record" class="Bool (strict)"("Value"=w1287) -> ()  [unwired: 2 in, 2 out]
              }
            }
            n486 = Bundle By Name(cluster=w1277, "tdms file"=w1263, "Record"=w1274) -> (w1276:T1)
          }
        }
      }
    }
  }
  n487 = Merge Errors(w22, w24) -> (w23:errorcluster)
  n488 = Unregister For Events(event registration refnum=w17) -> ()  [unwired: 1 in, 1 out]
  n489 = call "DestroyStandardEvents.vi"("error in"=w23, "standard events"=w16) -> ()  [unwired: 9 in, 1 out]
